vi "Write Sample Metadata.vi"(0 "File Path":path, 11 "Error In":errorcluster) -> (4 "File Path (Dup)":path, 8 "Canceled?":bool, 15 "Write Error":errorcluster)   [LabVIEW 2016]
uses:
  <vilib>/Utility/miscctls.llb/LVPointTypeDef.ctl
  Sampel Metadata Type Defs/Sample Metadata Full Data.ctl
  Sampel Metadata Type Defs/Sample Metadata Name Value Pair.ctl
  Sampel Metadata Type Defs/Sample Metadata Probe Data.ctl
  <vilib>/regexp/Match Regular Expression.xnode
  shell32.dll
panel:
  in  "Abort":bool
  in  "User Name":u16(ring) items=["Not Applicable", "-", "Add Item"]
  out "Current Path":string
  out "Last File Write Error":errorcluster
  in  "Dirty Quit":bool
  in  "Scavenger 06":u16(ring) items=["Not Applicable", "-", "Add Item"]
  in  "Scavenger 05":u16(ring) items=["Not Applicable", "-", "Add Item"]
  in  "Scavenger 04":u16(ring) items=["Not Applicable", "-", "Add Item"]
  in  "Scavenger 03":u16(ring) items=["Not Applicable", "-", "Add Item"]
  in  "Scavenger 02":u16(ring) items=["Not Applicable", "-", "Add Item"]
  in  "Scavenger 01":u16(ring) items=["Not Applicable", "-", "Add Item"]
  in  "Load Preset":bool
  in  "Sealant":u16(ring) items=["Not Applicable", "-", "Add Item"]
  in  "Sample Holder":u16(ring) items=["Not Applicable", "-", "Add Item"]
  in  "Preset Metadata":u16(ring) items=["None"]
  in  "Save New Preset":bool
  in  "Notes":string caption="Additional Notes (e.g. fixation info)"
  in  "Extra Tag 06":u16(ring) caption="Extra Tag" items=["Not Applicable", "-", "Add Item"]
  in  "Extra Tag 05":u16(ring) caption="Extra Tag" items=["Not Applicable", "-", "Add Item"]
  in  "Extra Tag 04":u16(ring) caption="Extra Tag" items=["Not Applicable", "-", "Add Item"]
  in  "Extra Tag 03":u16(ring) caption="Extra Tag" items=["Not Applicable", "-", "Add Item"]
  in  "Extra Tag 02":u16(ring) caption="Extra Tag" items=["Not Applicable", "-", "Add Item"]
  in  "Extra Tag 01":u16(ring) caption="Extra Tag" items=["Not Applicable", "-", "Add Item"]
  in  "Image Target 04":u16(ring) caption="Image Target" items=["Not Applicable", "-", "Add Item"]
  in  "Image Target 03":u16(ring) caption="Image Target" items=["Not Applicable", "-", "Add Item"]
  in  "Image Target 02":u16(ring) caption="Image Target" items=["Not Applicable", "-", "Add Item"]
  in  "Image Target 01":u16(ring) caption="Probe Target" items=["Not Applicable", "-", "Add Item"]
  in  "Buffer PH":dbl=1.0 caption="PH"
  in  "Buffer Type":u16(ring) items=["Not Applicable", "-", "Add Item"]
  in  "Probe Concentration 04":dbl=1.0 caption="Concentration"
  in  "Probe Concentration 03":dbl=1.0 caption="Concentration"
  in  "Probe Concentration 02":dbl=1.0 caption="Concentration"
  in  "Probe Concentration 01":dbl=1.0 caption="Concentration"
  in  "Probe Cat Num 04":u16(ring) caption="Probe Cat Num" items=["Not Applicable", "-", "Add Item"]
  in  "Probe Sub Type 04":u16(ring) caption="Probe Sub Type" items=["Not Applicable", "-", "Add Item"]
  in  "Probe Name 04":u16(ring) caption="Probe Name" items=["Not Applicable", "-", "Add Item"]
  in  "Probe 4":bool
  in  "Probe Cat Num 03":u16(ring) caption="Probe Cat Num" items=["Not Applicable", "-", "Add Item"]
  in  "Probe Cat Num 02":u16(ring) caption="Probe Cat Num" items=["Not Applicable", "-", "Add Item"]
  in  "Probe Cat Num 01":u16(ring) caption="Catalog Number" items=["Not Applicable", "-", "Add Item"]
  in  "Probe Sub Type 03":u16(ring) caption="Probe Sub Type" items=["Not Applicable", "-", "Add Item"]
  in  "Probe Sub Type 02":u16(ring) caption="Probe Sub Type" items=["Not Applicable", "-", "Add Item"]
  in  "Probe Sub Type 01":u16(ring) caption="Probe Sub Type" items=["Not Applicable", "-", "Add Item"]
  in  "Probe Name 03":u16(ring) caption="Probe Name" items=["Not Applicable", "-", "Add Item"]
  in  "Probe Name 02":u16(ring) caption="Probe Name" items=["Not Applicable", "-", "Add Item"]
  in  "Probe Name 01":u16(ring) caption="Probe Name" items=["Not Applicable", "-", "Add Item"]
  in  "Probe 3":bool
  in  "Probe 2":bool
  in  "Probe 1":bool
  in  "Sample Type Sub Types":u16(ring) caption="Sample Sub Type" items=["Not Applicable", "-", "Add Item"]
  in  "Sample Type":u16(ring) items=["Not Applicable", "-", "Add Item"]
  in  "Cancel":bool
  in  "Save":bool
  # "Sample Type"
  # "Sample Mounting"
  # "Buffer Information"
  # "Oxygen Scavenger Components"
  # "Probe Information"
  # "Probe Active"
  # "Additional Tags"
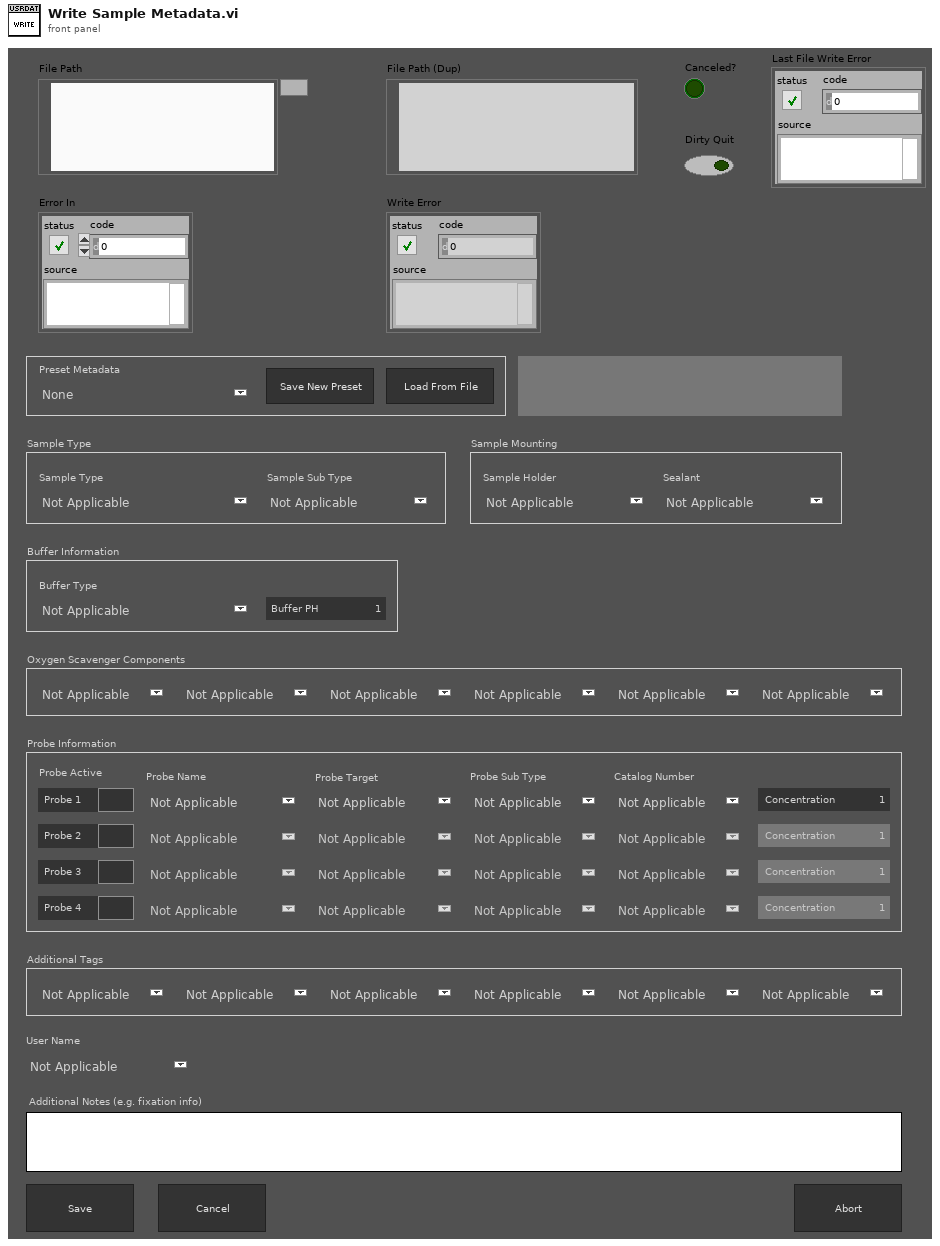
[diagram p1: front panel]
types:
  T1 = typedef "Sample Metadata Full Data.ctl" = cluster{"Sample Type":T2, "Sample Sub Type":T2, "Proble Data":T3[], "Buffer Type":T2, "Buffer PH":dbl, "Extra Tags":T2[], "Sample Holder":T2, "Sealant":T2, "Notes":string, "Preset Name":string, "Scavenger Tags":T2[], "User Name":T2}
  T2 = typedef "Sample Metadata Name Value Pair.ctl" = cluster{"String":string, "Value":u16}
  T3 = typedef "Sample Metadata Probe Data.ctl" = cluster{"Active?":bool, "Name":T2, "Target":T2, "Sub Type":T2, "Cat Number":T2, "Concentration":dbl}
  T4 = enum16{"Always On", "Always Off", "Off While Running"}
  T5 = typedef "LVPointTypeDef.ctl" = cluster{"Horizontal":i16, "Vertical":i16}
  T6 = enum8{"Enabled", "Disabled", "Disabled and Grayed Out"}
  T7 = typedef "LVRectTypeDef.ctl" = cluster{"Left":i16, "Top":i16, "Right":i16, "Bottom":i16}
  T8 = typedef "LVBoundsTypeDef.ctl" = cluster{"Width":u32, "Height":u32}
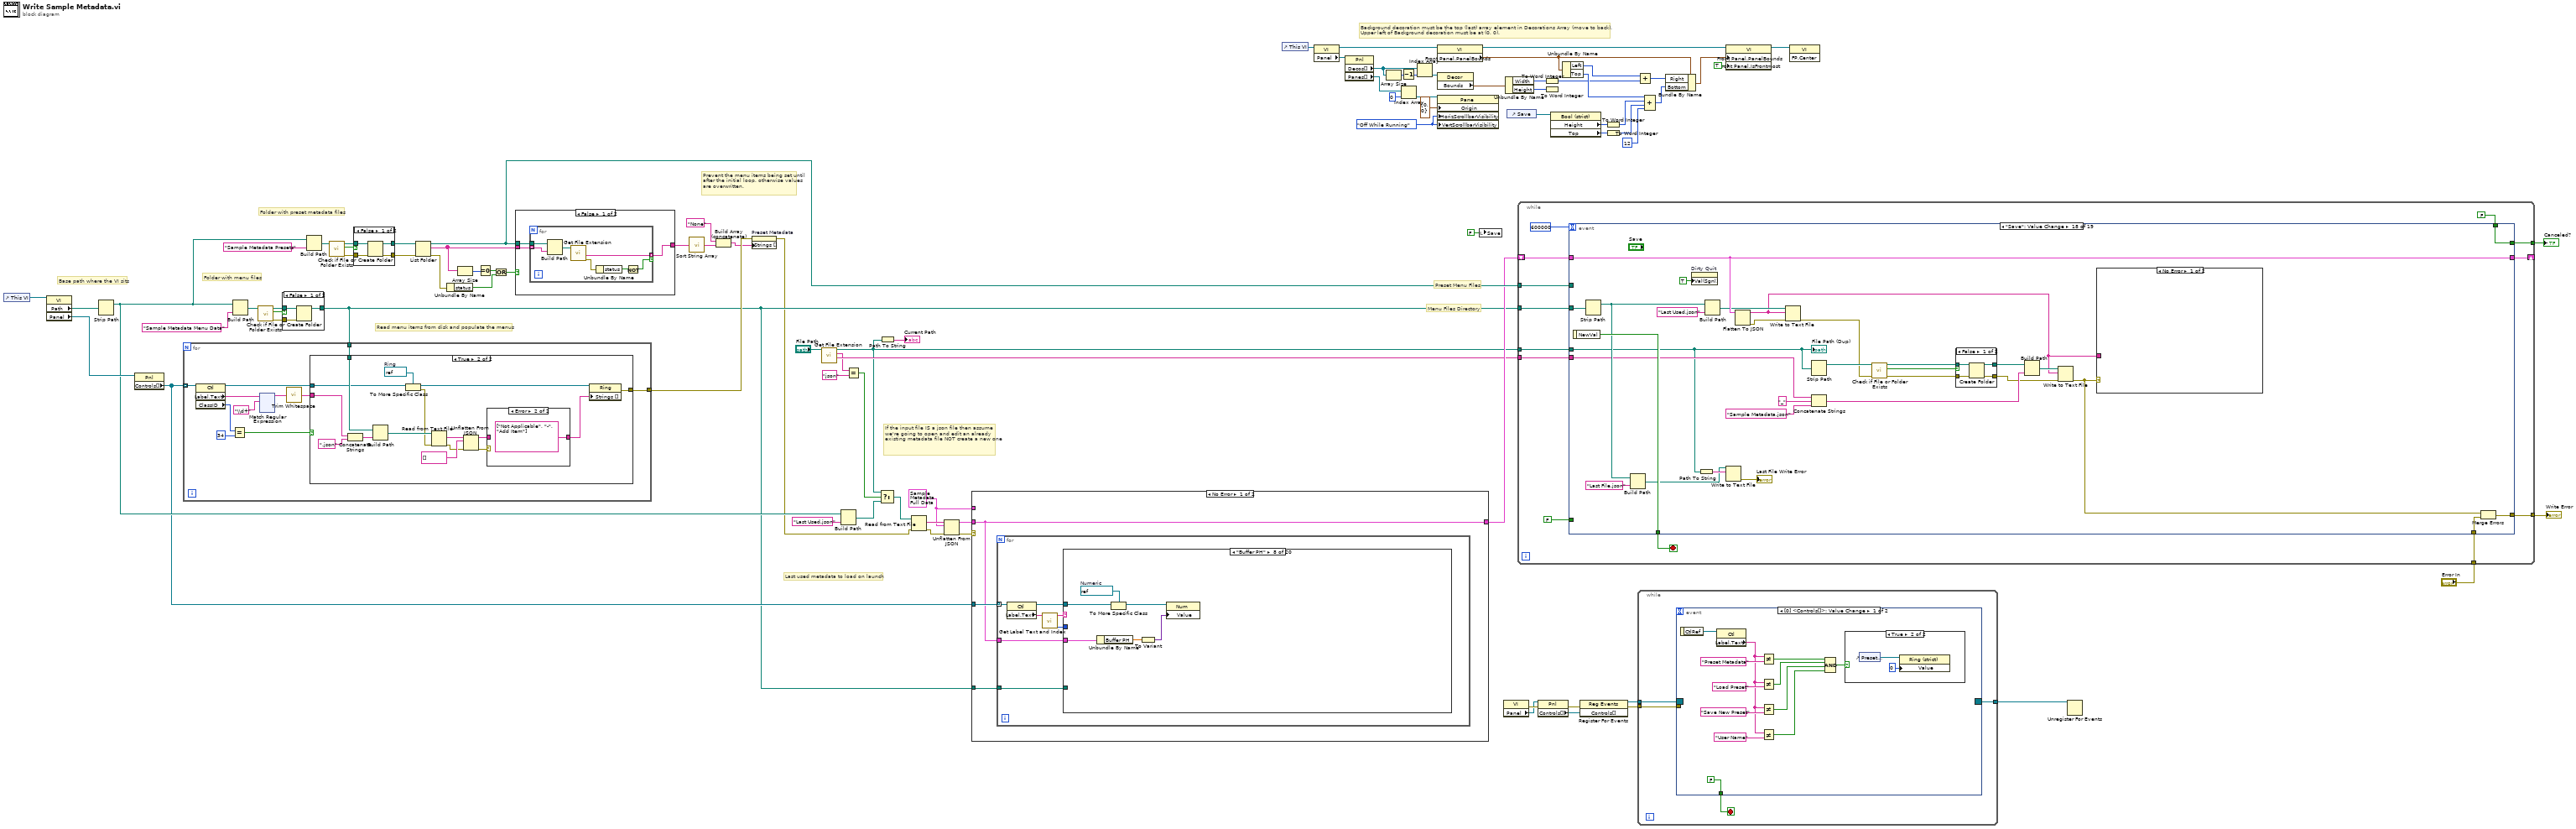
[diagram p0: block diagram]
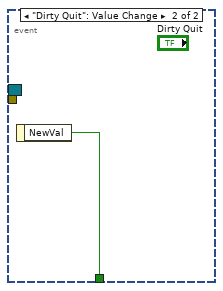
[diagram p3: hidden frame]
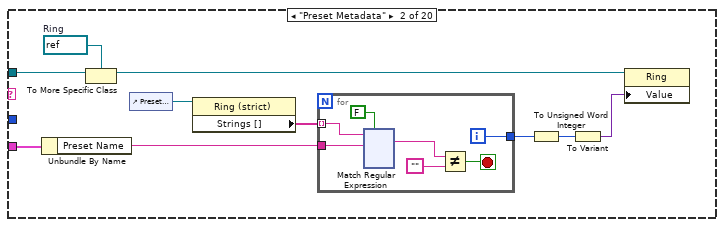
[diagram p5: hidden frame]
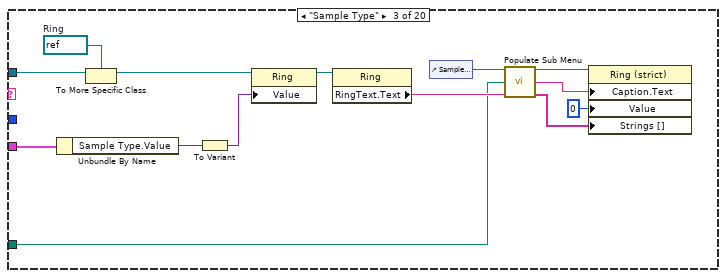
[diagram p6: hidden frame]
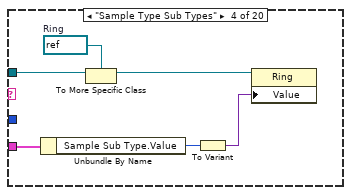
[diagram p7: hidden frame]
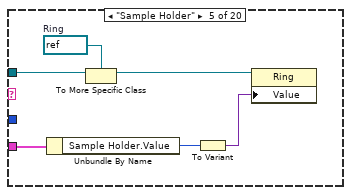
[diagram p8: hidden frame]
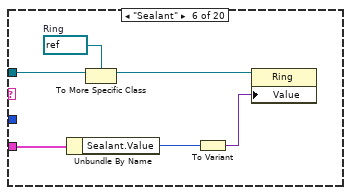
[diagram p9: hidden frame]
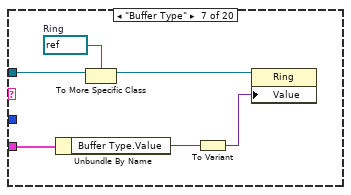
[diagram p10: hidden frame]
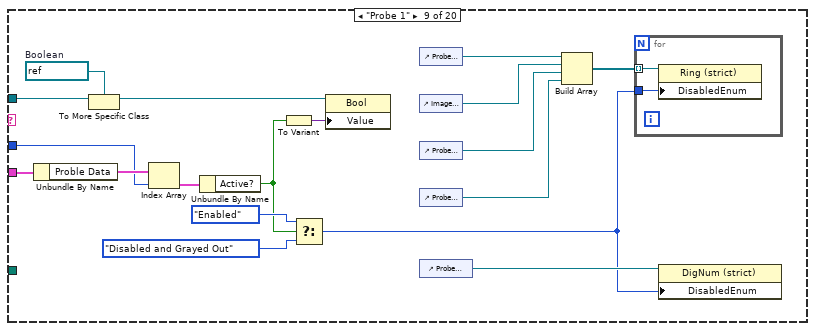
[diagram p11: hidden frame]
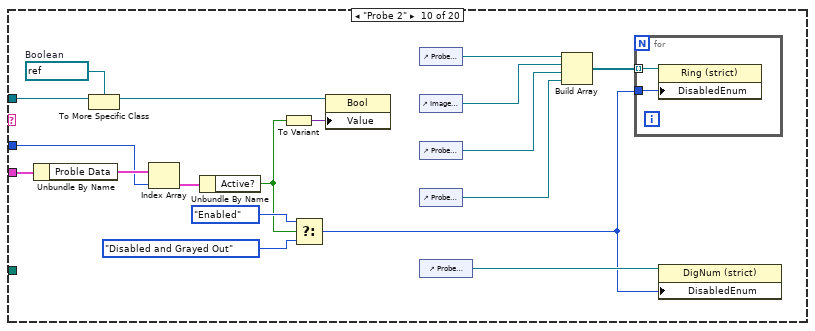
[diagram p12: hidden frame]
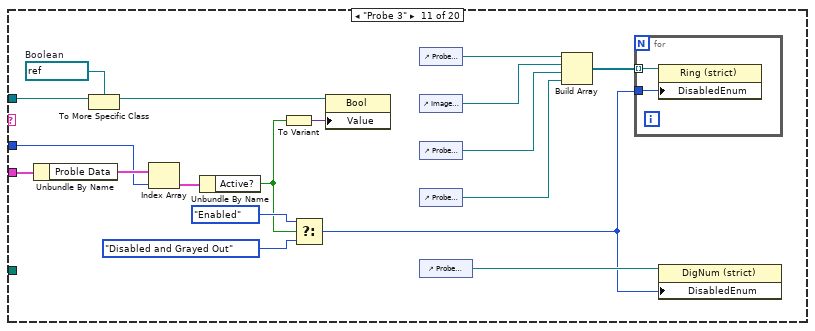
[diagram p13: hidden frame]
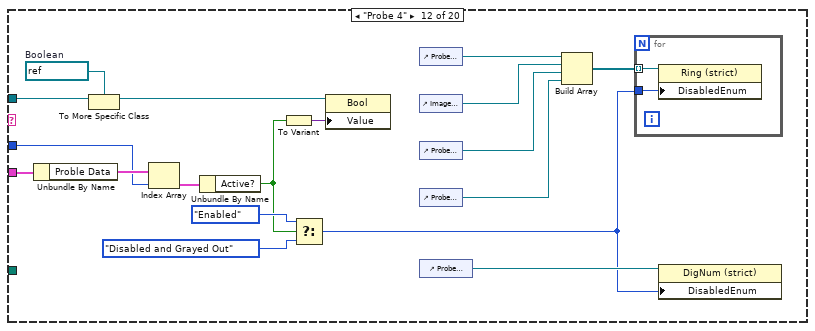
[diagram p14: hidden frame]
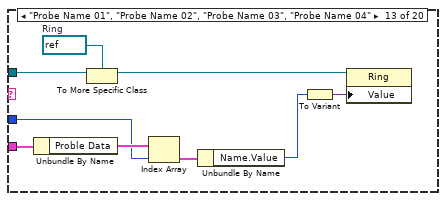
[diagram p15: hidden frame]
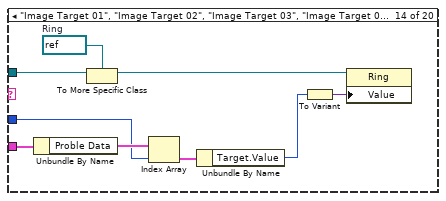
[diagram p16: hidden frame]
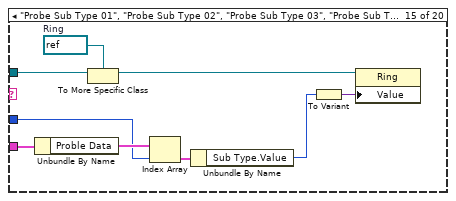
[diagram p17: hidden frame]
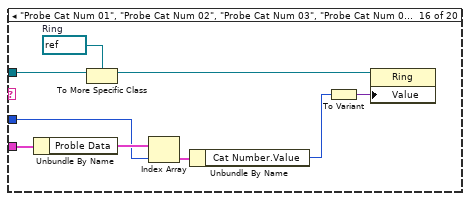
[diagram p18: hidden frame]
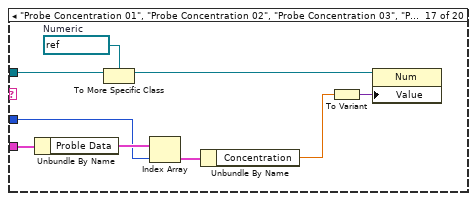
[diagram p19: hidden frame]
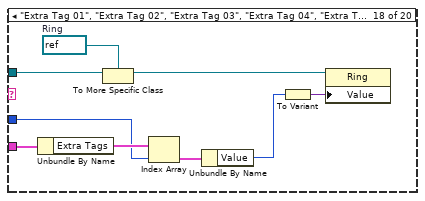
[diagram p20: hidden frame]
diagram:
  w30 = T1 {"Sample Type"={"String"="", "Value"=0}, "Sample Sub Type"={"String"="", "Value"=0}, "Proble Data"=[{"Active?"=FALSE, "Name"={"String"="", "Value"=0}, "Target"={"String"="", "Value"=0}, "Sub Type"={"String"="", "Value"=0}, "Cat Number"={"String"="", "Value"=0}, "Concentration"=0.0}, {"Active?"=FALSE, "Name"={"String"="", "Value"=0}, "Target"={"String"="", "Value"=0}, "Sub Type"={"String"="", "Value"=0}, "Cat Number"={"String"="", "Value"=0}, "Concentration"=0.0}, {"Active?"=FALSE, "Name"={"String"="", "Value"=0}, "Target"={"String"="", "Value"=0}, "Sub Type"={"String"="", "Value"=0}, "Cat Number"={"String"="", "Value"=0}, "Concentration"=0.0}, {"Active?"=FALSE, "Name"={"String"="", "Value"=0}, "Target"={"String"="", "Value"=0}, "Sub Type"={"String"="", "Value"=0}, "Cat Number"={"String"="", "Value"=0}, "Concentration"=0.0}], "Buffer Type"={"String"="", "Value"=0}, "Buffer PH"=0.0, "Extra Tags"=[{"String"="", "Value"=0}, {"String"="", "Value"=0}, {"String"="", "Value"=0}, {"String"="", "Value"=0}, {"String"="", "Value"=0}, {"String"="", "Value"=0}], "Sample Holder"={"String"="", "Value"=0}, "Sealant"={"String"="", "Value"=0}, "Notes"="", "Preset Name"="", "Scavenger Tags"=[{"String"="", "Value"=0}, {"String"="", "Value"=0}, {"String"="", "Value"=0}, {"String"="", "Value"=0}, {"String"="", "Value"=0}, {"String"="", "Value"=0}], "User Name"={"String"="", "Value"=0}} ("Sample Metadata")
  w72 = T4."Off While Running" ("Vertical Scrollbar Visibility")
  # "If the input file IS a json file then assume we're going to open and edit an already existing metadata file NOT create a new one"
  # "Last used metadata to load on launch"
  # "Preset Menu Files"
  # "Menu Files Directory"
  # "Prevent the menu items being set until after the initial loop, otherwise values are overwritten."
  # "Folder with preset metadata files"
  # "Folder with menu files"
  # "Read menu items from disk and populate the menus"
  # "Base path where the VI sits"
  # "Background decoration must be the top (last) array element in Decorations Array (move to back).\nUpper left of Background decoration must be at (0, 0)."
  n1 = control-ref of="This VI"() -> (w58:refnum<vi>)
  n2 = property class="VI"(reference=w58) -> ("Path"=w35:path, "Panel"=w56:refnum<vi>)  [unwired: 1 in, 2 out]
  n3 = Strip Path(path=w35) -> (stripped path=w34:path)  [unwired: 1 out]
  n4 = property class="Pnl"(reference=w56) -> ("Controls[]"=w29:refnum<vi>[])  [unwired: 1 in, 2 out]
  n5 = Build Path(base path=w34, name or relative path="Sample Metadata Menu Data") -> (appended path=w54:path)
  n6 = call <vilib>:"Check if File or Folder Exists.vi"("path"=w54) -> ("error out"=w39:errorcluster, "file or folder exists?"=w52:bool, "dup path"=w53:path)  [unwired: 8 in]
  n7 = case shown="False" w52 {
    tunnel: w53 -> [w92 w93]
    tunnel: [w91 w93] -> w27
    tunnel: w39 -> [w90 _]
    frame False {
      n8 = Create Folder(path (use dialog)=w92, error in=w90) -> (created path=w91:path)  [unwired: 1 in, 2 out]
    }
    frame True {
    }
  }
  n9 = for {
    tunnel: w29 -> [w104] mode=indexing
    tunnel: w27 -> [w100]
    tunnel: [w94] -> w38
    n10 = property class="Ctl"(reference=w104) -> (reference out=w102:refnum<vi>, "Label.Text"=w97:string, "ClassID"=w101:u32)  [unwired: 1 in, 1 out]
    n11 = Equal?(x=w101, y=u32 34) -> (x = y?=w103:bool)
    n12 = xnode "Match Regular Expression"("input string"=w97, "regular expression"="\\d+") -> ("before match"=w99:string)  [unwired: 4 in, 4 out]
    n13 = call <vilib>:"Trim Whitespace.vi"("string"=w99) -> ("trimmed string"=w96:string)  [unwired: 1 in]
    n14 = case shown="True" w103 {
      tunnel: w102 -> [_ w225]
      tunnel: w96 -> [_ w233]
      tunnel: w100 -> [_ w232]
      tunnel: [errorcluster {"status"=FALSE, "code"=0, "source"=""} ("error out") w220] -> w94
      frame False {
      }
      frame True {
        w224 = refnum<vi> refnum  # Ring
        n15 = Concatenate Strings(w233, ".json") -> (w234:string)
        n16 = Build Path(base path=w232, name or relative path=w234) -> (appended path=w231:path)
        n17 = To More Specific Class(target class=w224, reference=w225) -> (specific class reference=w223:refnum<vi>, error out=w221:errorcluster)  [unwired: 1 in]
        n18 = Read from Text File(file (use dialog)=w231, error in=w221) -> (text=w230:string, error out=w228:errorcluster)  [unwired: 2 in, 2 out]
        n19 = Unflatten From JSON(JSON string=w230, type and defaults=string[] [], error in (no error)=w228) -> (value=w226:string[], error out=w227:errorcluster)  [unwired: 4 in]
        n20 = case shown="Error" w227 {
          tunnel: w226 -> [w236 _]
          tunnel: [w236 string[] ["Not Applicable", "-", "Add Item"]] -> w222
          frame No Error {
          }
          frame Error {
          }
        }
        n21 = property class="Ring"(reference=w223, "Strings []"=w222) -> (error out=w220:errorcluster)  [unwired: 1 in, 1 out]
      }
    }
  }
  n22 = Build Path(base path=w34, name or relative path="Sample Metadata Presets") -> (appended path=w49:path)
  n23 = call <vilib>:"Check if File or Folder Exists.vi"("path"=w49) -> ("error out"=w41:errorcluster, "file or folder exists?"=w51:bool, "dup path"=w50:path)  [unwired: 8 in]
  n24 = case shown="False" w51 {
    tunnel: w50 -> [w241 w243]
    tunnel: [w240 w243] -> w48
    tunnel: w41 -> [w239 w242]
    tunnel: [w238 w242] -> w40
    frame False {
      n25 = Create Folder(path (use dialog)=w241, error in=w239) -> (created path=w240:path, error out=w238:errorcluster)  [unwired: 1 in, 1 out]
    }
    frame True {
    }
  }
  n26 = List Folder(path=w48, error in=w40) -> (path out=w37:path, filenames=w46:string[], error out=w47:errorcluster)  [unwired: 2 in, 1 out]
  n27 = Unbundle By Name(w47) -> ("status"=w43:bool)
  n28 = Array Size(array=w46) -> (size(s)=w45:i32)
  n29 = Equal To 0?(x=w45) -> (x = 0?=w44:bool)
  n30 = Or(x=w44, y=w43) -> (x .or. y?=w42:bool)
  n31 = case shown="False" w42 {
    tunnel: w46 -> [w246 _]
    tunnel: [w244 string[] []] -> w23
    tunnel: w37 -> [w245 _]
    frame False {
      n32 = for {
        tunnel: w246 -> [w252] mode=indexing
        tunnel: w245 -> [w253]
        tunnel: [w250] -> w244 mode=indexing if=w247
        n33 = Build Path(base path=w253, name or relative path=w252) -> (appended path=w251:path)
        n34 = call <vilib>:"Get File Extension.vi"("file"=w251) -> ("error out"=w249:errorcluster, "filename without extension"=w250:string)  [unwired: 6 in, 3 out]
        n35 = Unbundle By Name(w249) -> ("status"=w248:bool)
        n36 = Not(x=w248) -> (.not. x?=w247:bool)
      }
    }
    frame True {
    }
  }
  n37 = call "Sort String Array.vi"("Array of String"=w23) -> ("Sorted Array"=w22:string[])  [unwired: 14 in]
  n38 = Build Array (concatenate)("None", w22) -> (w20:string[])
  n39 = property on="Preset Metadata" class="Ring (strict)"(error in=w38, "Strings []"=w20) -> (error out=w19:errorcluster)  [unwired: 1 in, 1 out]
  n40 = call <vilib>:"Get File Extension.vi"("file"="File Path") -> ("filename without extension"=w9:string, "lowercase file extension"=w8:string, "dup file"=w3:path)  [unwired: 6 in, 2 out]
  n41 = Build Path(base path=w34, name or relative path="Last Used.json") -> (appended path=w5:path)
  n42 = Equal?(x=w8, y="json") -> (x = y?=w6:bool)
  n43 = Select(t=w3, s=w6, f=w5) -> (s? t:f=w4:path)
  n44 = Path To String(path=w3) -> (string=→"Current Path":string)
  n45 = Read from Text File(file (use dialog)=w4, error in=w19) -> (text=w33:string, error out=w18:errorcluster)  [unwired: 2 in, 2 out]
  n46 = Unflatten From JSON(JSON string=w33, type and defaults=w30, error in (no error)=w18) -> (value=w31:T1, error out=w32:errorcluster)  [unwired: 4 in]
  n47 = case shown="No Error" w32 {
    tunnel: [w255 w597] -> w28
    tunnel: w29 -> [w257 _]
    tunnel: w27 -> [w256 w589]
    tunnel: w31 -> [w255 _]
    tunnel: w30 -> [_ w597]
    frame No Error {
      n48 = for {
        tunnel: w257 -> [w264] mode=indexing
        tunnel: w255 -> [w262]
        tunnel: w256 -> [w261]
        n49 = property class="Ctl"(reference=w264) -> (reference out=w263:refnum<vi>, "Label.Text"=w260:string)  [unwired: 1 in, 1 out]
        n50 = call "Get Label Text and Index.vi"("Label Text and Index"=w260) -> ("Label Text and Index (Dup)"=w259:string, "Index"=w258:i32)  [unwired: 12 in, 1 out]
        n51 = case shown="\"Buffer PH\"" w259 {
          tunnel: w263 -> [_ w273 w408 w414 w420 w426 w432 w438 w453 w473 w493 w513 w525 w534 w543 w552 w561 w570 w579 w585]
          tunnel: w262 -> [_ w271 w406 w412 w418 w424 w430 w436 w457 w477 w497 w517 w528 w537 w546 w555 w564 w573 w582 w584]
          tunnel: w261 -> [_ _ w396 _ _ _ _ _ _ _ _ _ _ _ _ _ _ _ _ _]
          tunnel: w258 -> [_ _ _ _ _ _ _ _ w440 w460 w480 w500 w520 w529 w538 w547 w556 w565 w574 _]
          frame Default {
          }
          frame "Preset Metadata" {
            w274 = refnum<vi> refnum  # Ring
            n52 = Unbundle By Name(w271) -> ("Preset Name"=w266:string)
            n53 = To More Specific Class(target class=w274, reference=w273) -> (specific class reference=w272:refnum<vi>)  [unwired: 1 in, 1 out]
            n54 = control-ref of="Preset Metadata"() -> (w268:refnum<vi>)
            n55 = property class="Ring (strict)"(reference=w268) -> ("Strings []"=w269:string[])  [unwired: 1 in, 2 out]
            n56 = for {
              tunnel: w266 -> [w281]
              tunnel: w269 -> [w279] mode=indexing
              tunnel: [w275] -> w267
              i -> [w275]
              stop <- w278 stop-if-true
              n57 = xnode "Match Regular Expression"("input string"=w279, "regular expression"=w281, "ignore case? (F)"=FALSE) -> ("whole match"=w277:string)  [unwired: 3 in, 4 out]
              n58 = Not Equal?(x=w277, y="") -> (x != y?=w278:bool)
            }
            n59 = To Unsigned Word Integer(number=w267) -> (unsigned 16bit integer=w265:u16)
            n60 = To Variant(anything=w265) -> (Variant=w270:variant)
            n61 = property class="Ring"(reference=w272, "Value"=w270) -> ()  [unwired: 1 in, 2 out]
          }
          frame "Sample Type" {
            w409 = refnum<vi> refnum  # Ring
            n62 = Unbundle By Name(w406) -> ("Sample Type.Value"=w405:u16)
            n63 = To More Specific Class(target class=w409, reference=w408) -> (specific class reference=w407:refnum<vi>)  [unwired: 1 in, 1 out]
            n64 = To Variant(anything=w405) -> (Variant=w404:variant)
            n65 = property class="Ring"(reference=w407, "Value"=w404) -> (reference out=w403:refnum<vi>)  [unwired: 1 in, 1 out]
            n66 = property class="Ring"(reference=w403) -> ("RingText.Text"=w397:string)  [unwired: 1 in, 2 out]
            n67 = control-ref of="Sample Type Sub Types"() -> (w401:refnum<vi>)
            n68 = call "Populate Sub Menu.vi"("Sample Type Sub Types"=w401, "Base Path"=w396, "Ring Text"=w397) -> ("Sample Type Sub Types (Dup)"=w400:refnum<vi>, "Caption Text"=w399:string, "Menu Items"=w398:string[])  [unwired: 10 in]
            n69 = property class="Ring (strict)"(reference=w400, "Caption.Text"=w399, "Value"=u16 0, "Strings []"=w398) -> ()  [unwired: 1 in, 2 out]
          }
          frame "Sample Type Sub Types" {
            w415 = refnum<vi> refnum  # Ring
            n70 = Unbundle By Name(w412) -> ("Sample Sub Type.Value"=w411:u16)
            n71 = To More Specific Class(target class=w415, reference=w414) -> (specific class reference=w413:refnum<vi>)  [unwired: 1 in, 1 out]
            n72 = To Variant(anything=w411) -> (Variant=w410:variant)
            n73 = property class="Ring"(reference=w413, "Value"=w410) -> ()  [unwired: 1 in, 2 out]
          }
          frame "Sample Holder" {
            w421 = refnum<vi> refnum  # Ring
            n74 = Unbundle By Name(w418) -> ("Sample Holder.Value"=w417:u16)
            n75 = To More Specific Class(target class=w421, reference=w420) -> (specific class reference=w419:refnum<vi>)  [unwired: 1 in, 1 out]
            n76 = To Variant(anything=w417) -> (Variant=w416:variant)
            n77 = property class="Ring"(reference=w419, "Value"=w416) -> ()  [unwired: 1 in, 2 out]
          }
          frame "Sealant" {
            w427 = refnum<vi> refnum  # Ring
            n78 = Unbundle By Name(w424) -> ("Sealant.Value"=w423:u16)
            n79 = To More Specific Class(target class=w427, reference=w426) -> (specific class reference=w425:refnum<vi>)  [unwired: 1 in, 1 out]
            n80 = To Variant(anything=w423) -> (Variant=w422:variant)
            n81 = property class="Ring"(reference=w425, "Value"=w422) -> ()  [unwired: 1 in, 2 out]
          }
          frame "Buffer Type" {
            w433 = refnum<vi> refnum  # Ring
            n82 = Unbundle By Name(w430) -> ("Buffer Type.Value"=w429:u16)
            n83 = To More Specific Class(target class=w433, reference=w432) -> (specific class reference=w431:refnum<vi>)  [unwired: 1 in, 1 out]
            n84 = To Variant(anything=w429) -> (Variant=w428:variant)
            n85 = property class="Ring"(reference=w431, "Value"=w428) -> ()  [unwired: 1 in, 2 out]
          }
          frame "Buffer PH" {
            w439 = refnum<vi> refnum  # Numeric
            n86 = Unbundle By Name(w436) -> ("Buffer PH"=w435:dbl)
            n87 = To More Specific Class(target class=w439, reference=w438) -> (specific class reference=w437:refnum<vi>)  [unwired: 1 in, 1 out]
            n88 = To Variant(anything=w435) -> (Variant=w434:variant)
            n89 = property class="Num"(reference=w437, "Value"=w434) -> ()  [unwired: 1 in, 2 out]
          }
          frame "Probe 1" {
            w454 = refnum<vi> refnum  # Boolean
            n90 = Unbundle By Name(w457) -> ("Proble Data"=w456:T3[])
            n91 = To More Specific Class(target class=w454, reference=w453) -> (specific class reference=w452:refnum<vi>)  [unwired: 1 in, 1 out]
            n92 = Index Array(array=w456, index=w440) -> (element=w455:T3)
            n93 = Unbundle By Name(w455) -> ("Active?"=w442:bool)
            n94 = To Variant(anything=w442) -> (Variant=w451:variant)
            n95 = Select(t=T6."Enabled" ("Disabled"), s=w442, f=T6."Disabled and Grayed Out" ("Disabled")) -> (s? t:f=w441:T6)
            n96 = property class="Bool"(reference=w452, "Value"=w451) -> ()  [unwired: 1 in, 2 out]
            n97 = control-ref of="Probe Name 01"() -> (w447:refnum<vi>)
            n98 = control-ref of="Image Target 01"() -> (w448:refnum<vi>)
            n99 = control-ref of="Probe Sub Type 01"() -> (w449:refnum<vi>)
            n100 = control-ref of="Probe Cat Num 01"() -> (w450:refnum<vi>)
            n101 = control-ref of="Probe Concentration 01"() -> (w445:refnum<vi>)
            n102 = Build Array(w447, w448, w449, w450) -> (w446:refnum<vi>[])
            n103 = for {
              tunnel: w446 -> [w459] mode=indexing
              tunnel: w441 -> [w458]
              n104 = property class="Ring (strict)"(reference=w459, "DisabledEnum"=w458) -> ()  [unwired: 1 in, 2 out]
            }
            n105 = property class="DigNum (strict)"(reference=w445, "DisabledEnum"=w441) -> ()  [unwired: 1 in, 2 out]
          }
          frame "Probe 2" {
            w474 = refnum<vi> refnum  # Boolean
            n106 = Unbundle By Name(w477) -> ("Proble Data"=w476:T3[])
            n107 = To More Specific Class(target class=w474, reference=w473) -> (specific class reference=w472:refnum<vi>)  [unwired: 1 in, 1 out]
            n108 = Index Array(array=w476, index=w460) -> (element=w475:T3)
            n109 = Unbundle By Name(w475) -> ("Active?"=w462:bool)
            n110 = To Variant(anything=w462) -> (Variant=w471:variant)
            n111 = Select(t=T6."Enabled" ("Disabled"), s=w462, f=T6."Disabled and Grayed Out" ("Disabled")) -> (s? t:f=w461:T6)
            n112 = property class="Bool"(reference=w472, "Value"=w471) -> ()  [unwired: 1 in, 2 out]
            n113 = control-ref of="Probe Name 02"() -> (w467:refnum<vi>)
            n114 = control-ref of="Image Target 02"() -> (w468:refnum<vi>)
            n115 = control-ref of="Probe Sub Type 02"() -> (w469:refnum<vi>)
            n116 = control-ref of="Probe Cat Num 02"() -> (w470:refnum<vi>)
            n117 = control-ref of="Probe Concentration 02"() -> (w465:refnum<vi>)
            n118 = Build Array(w467, w468, w469, w470) -> (w466:refnum<vi>[])
            n119 = for {
              tunnel: w466 -> [w479] mode=indexing
              tunnel: w461 -> [w478]
              n120 = property class="Ring (strict)"(reference=w479, "DisabledEnum"=w478) -> ()  [unwired: 1 in, 2 out]
            }
            n121 = property class="DigNum (strict)"(reference=w465, "DisabledEnum"=w461) -> ()  [unwired: 1 in, 2 out]
          }
          frame "Probe 3" {
            w494 = refnum<vi> refnum  # Boolean
            n122 = Unbundle By Name(w497) -> ("Proble Data"=w496:T3[])
            n123 = To More Specific Class(target class=w494, reference=w493) -> (specific class reference=w492:refnum<vi>)  [unwired: 1 in, 1 out]
            n124 = Index Array(array=w496, index=w480) -> (element=w495:T3)
            n125 = Unbundle By Name(w495) -> ("Active?"=w482:bool)
            n126 = To Variant(anything=w482) -> (Variant=w491:variant)
            n127 = Select(t=T6."Enabled" ("Disabled"), s=w482, f=T6."Disabled and Grayed Out" ("Disabled")) -> (s? t:f=w481:T6)
            n128 = property class="Bool"(reference=w492, "Value"=w491) -> ()  [unwired: 1 in, 2 out]
            n129 = control-ref of="Probe Name 03"() -> (w487:refnum<vi>)
            n130 = control-ref of="Image Target 03"() -> (w488:refnum<vi>)
            n131 = control-ref of="Probe Sub Type 03"() -> (w489:refnum<vi>)
            n132 = control-ref of="Probe Cat Num 03"() -> (w490:refnum<vi>)
            n133 = control-ref of="Probe Concentration 03"() -> (w485:refnum<vi>)
            n134 = Build Array(w487, w488, w489, w490) -> (w486:refnum<vi>[])
            n135 = for {
              tunnel: w486 -> [w499] mode=indexing
              tunnel: w481 -> [w498]
              n136 = property class="Ring (strict)"(reference=w499, "DisabledEnum"=w498) -> ()  [unwired: 1 in, 2 out]
            }
            n137 = property class="DigNum (strict)"(reference=w485, "DisabledEnum"=w481) -> ()  [unwired: 1 in, 2 out]
          }
          frame "Probe 4" {
            w514 = refnum<vi> refnum  # Boolean
            n138 = Unbundle By Name(w517) -> ("Proble Data"=w516:T3[])
            n139 = To More Specific Class(target class=w514, reference=w513) -> (specific class reference=w512:refnum<vi>)  [unwired: 1 in, 1 out]
            n140 = Index Array(array=w516, index=w500) -> (element=w515:T3)
            n141 = Unbundle By Name(w515) -> ("Active?"=w502:bool)
            n142 = To Variant(anything=w502) -> (Variant=w511:variant)
            n143 = Select(t=T6."Enabled" ("Disabled"), s=w502, f=T6."Disabled and Grayed Out" ("Disabled")) -> (s? t:f=w501:T6)
            n144 = property class="Bool"(reference=w512, "Value"=w511) -> ()  [unwired: 1 in, 2 out]
            n145 = control-ref of="Probe Name 04"() -> (w507:refnum<vi>)
            n146 = control-ref of="Image Target 04"() -> (w508:refnum<vi>)
            n147 = control-ref of="Probe Sub Type 04"() -> (w509:refnum<vi>)
            n148 = control-ref of="Probe Cat Num 04"() -> (w510:refnum<vi>)
            n149 = control-ref of="Probe Concentration 04"() -> (w505:refnum<vi>)
            n150 = Build Array(w507, w508, w509, w510) -> (w506:refnum<vi>[])
            n151 = for {
              tunnel: w506 -> [w519] mode=indexing
              tunnel: w501 -> [w518]
              n152 = property class="Ring (strict)"(reference=w519, "DisabledEnum"=w518) -> ()  [unwired: 1 in, 2 out]
            }
            n153 = property class="DigNum (strict)"(reference=w505, "DisabledEnum"=w501) -> ()  [unwired: 1 in, 2 out]
          }
          frame "Probe Name 01", "Probe Name 02", "Probe Name 03", "Probe Name 04" {
            w521 = refnum<vi> refnum  # Ring
            n154 = Unbundle By Name(w528) -> ("Proble Data"=w527:T3[])
            n155 = To More Specific Class(target class=w521, reference=w525) -> (specific class reference=w524:refnum<vi>)  [unwired: 1 in, 1 out]
            n156 = Index Array(array=w527, index=w520) -> (element=w526:T3)
            n157 = Unbundle By Name(w526) -> ("Name.Value"=w522:u16)
            n158 = To Variant(anything=w522) -> (Variant=w523:variant)
            n159 = property class="Ring"(reference=w524, "Value"=w523) -> ()  [unwired: 1 in, 2 out]
          }
          frame "Image Target 01", "Image Target 02", "Image Target 03", "Image Target 04" {
            w530 = refnum<vi> refnum  # Ring
            n160 = Unbundle By Name(w537) -> ("Proble Data"=w536:T3[])
            n161 = To More Specific Class(target class=w530, reference=w534) -> (specific class reference=w533:refnum<vi>)  [unwired: 1 in, 1 out]
            n162 = Index Array(array=w536, index=w529) -> (element=w535:T3)
            n163 = Unbundle By Name(w535) -> ("Target.Value"=w531:u16)
            n164 = To Variant(anything=w531) -> (Variant=w532:variant)
            n165 = property class="Ring"(reference=w533, "Value"=w532) -> ()  [unwired: 1 in, 2 out]
          }
          frame "Probe Sub Type 01", "Probe Sub Type 02", "Probe Sub Type 03", "Probe Sub Type 04" {
            w539 = refnum<vi> refnum  # Ring
            n166 = Unbundle By Name(w546) -> ("Proble Data"=w545:T3[])
            n167 = To More Specific Class(target class=w539, reference=w543) -> (specific class reference=w542:refnum<vi>)  [unwired: 1 in, 1 out]
            n168 = Index Array(array=w545, index=w538) -> (element=w544:T3)
            n169 = Unbundle By Name(w544) -> ("Sub Type.Value"=w540:u16)
            n170 = To Variant(anything=w540) -> (Variant=w541:variant)
            n171 = property class="Ring"(reference=w542, "Value"=w541) -> ()  [unwired: 1 in, 2 out]
          }
          frame "Probe Cat Num 01", "Probe Cat Num 02", "Probe Cat Num 03", "Probe Cat Num 04" {
            w548 = refnum<vi> refnum  # Ring
            n172 = Unbundle By Name(w555) -> ("Proble Data"=w554:T3[])
            n173 = To More Specific Class(target class=w548, reference=w552) -> (specific class reference=w551:refnum<vi>)  [unwired: 1 in, 1 out]
            n174 = Index Array(array=w554, index=w547) -> (element=w553:T3)
            n175 = Unbundle By Name(w553) -> ("Cat Number.Value"=w549:u16)
            n176 = To Variant(anything=w549) -> (Variant=w550:variant)
            n177 = property class="Ring"(reference=w551, "Value"=w550) -> ()  [unwired: 1 in, 2 out]
          }
          frame "Probe Concentration 01", "Probe Concentration 02", "Probe Concentration 03", "Probe Concentration 04" {
            w557 = refnum<vi> refnum  # Numeric
            n178 = Unbundle By Name(w564) -> ("Proble Data"=w563:T3[])
            n179 = To More Specific Class(target class=w557, reference=w561) -> (specific class reference=w560:refnum<vi>)  [unwired: 1 in, 1 out]
            n180 = Index Array(array=w563, index=w556) -> (element=w562:T3)
            n181 = Unbundle By Name(w562) -> ("Concentration"=w558:dbl)
            n182 = To Variant(anything=w558) -> (Variant=w559:variant)
            n183 = property class="Num"(reference=w560, "Value"=w559) -> ()  [unwired: 1 in, 2 out]
          }
          frame "Extra Tag 01", "Extra Tag 02", "Extra Tag 03", "Extra Tag 04", "Extra Tag 05", "Extra Tag 06" {
            w566 = refnum<vi> refnum  # Ring
            n184 = Unbundle By Name(w573) -> ("Extra Tags"=w572:T2[])
            n185 = To More Specific Class(target class=w566, reference=w570) -> (specific class reference=w569:refnum<vi>)  [unwired: 1 in, 1 out]
            n186 = Index Array(array=w572, index=w565) -> (element=w571:T2)
            n187 = Unbundle By Name(w571) -> ("Value"=w567:u16)
            n188 = To Variant(anything=w567) -> (Variant=w568:variant)
            n189 = property class="Ring"(reference=w569, "Value"=w568) -> ()  [unwired: 1 in, 2 out]
          }
          frame "Scavenger 01", "Scavenger 02", "Scavenger 03", "Scavenger 04", "Scavenger 05", "Scavenger 06" {
            w575 = refnum<vi> refnum  # Ring
            n190 = Unbundle By Name(w582) -> ("Scavenger Tags"=w581:T2[])
            n191 = To More Specific Class(target class=w575, reference=w579) -> (specific class reference=w578:refnum<vi>)  [unwired: 1 in, 1 out]
            n192 = Index Array(array=w581, index=w574) -> (element=w580:T2)
            n193 = Unbundle By Name(w580) -> ("Value"=w576:u16)
            n194 = To Variant(anything=w576) -> (Variant=w577:variant)
            n195 = property class="Ring"(reference=w578, "Value"=w577) -> ()  [unwired: 1 in, 2 out]
          }
          frame "Notes" {
            w586 = refnum<vi> refnum  # String
            n196 = Unbundle By Name(w584) -> ("Notes"=w583:string)
            n197 = To More Specific Class(target class=w586, reference=w585) -> (specific class reference=w587:refnum<vi>)  [unwired: 1 in, 1 out]
            n198 = property class="Str"(reference=w587, "Value"=w583) -> ()  [unwired: 1 in, 2 out]
          }
        }
      }
    }
    frame Error {
      # "In the unlikely event that there is no \"Last Used.json\" file but there are sample sub type files we still want to load the sub type menu items"
      n199 = control-ref of="Sample Type"() -> (w590:refnum<vi>)
      n200 = property class="Ring (strict)"(reference=w590) -> (error out=w588:errorcluster, "RingText.Text"=w591:string)  [unwired: 1 in, 1 out]
      n201 = control-ref of="Sample Type Sub Types"() -> (w595:refnum<vi>)
      n202 = call "Populate Sub Menu.vi"("Sample Type Sub Types"=w595, "Base Path"=w589, "Ring Text"=w591) -> ("Sample Type Sub Types (Dup)"=w594:refnum<vi>, "Caption Text"=w593:string, "Menu Items"=w592:string[])  [unwired: 10 in]
      n203 = property class="Ring (strict)"(reference=w594, error in=w588, "Caption.Text"=w593, "Value"=u16 0, "Strings []"=w592) -> ()  [unwired: 2 out]
    }
  }
  n204 = control-ref of="This VI"() -> (w64:refnum<vi>)
  n205 = property class="VI"(reference=w64) -> (reference out=w73:refnum<vi>, "Panel"=w65:refnum<vi>)  [unwired: 1 in, 1 out]
  n206 = property class="Pnl"(reference=w65) -> ("Decos[]"=w63:refnum<vi>[], "Panes[]"=w69:refnum<vi>[])  [unwired: 1 in, 2 out]
  n207 = Array Size(array=w63) -> (size(s)=w61:i32)
  n208 = Decrement(x=w61) -> (x-1=w62:i32)
  n209 = Index Array(array=w69, index=0) -> (element=w68:refnum<vi>)
  n210 = Index Array(array=w63, index=w62) -> (element=w71:refnum<vi>)
  n211 = property class="VI"(reference=w73) -> (reference out=w75:refnum<vi>, "Front Panel.PanelBounds"=w76:T7)  [unwired: 1 in, 1 out]
  n212 = property class="Decor"(reference=w71) -> ("Bounds"=w74:T8)  [unwired: 1 in, 2 out]
  n213 = property class="Pane"(reference=w68, "Origin"=T5 {"Horizontal"=0, "Vertical"=0}, "HorizScrollbarVisibility"=w72, "VertScrollbarVisibility"=w72) -> ()  [unwired: 1 in, 2 out]
  n214 = local write "Save"(FALSE ("Save")) -> ()
  n215 = property class="VI"() -> (error out=w17:errorcluster, "Panel"=w16:refnum<vi>)  [unwired: 2 in, 1 out]
  n216 = Unbundle By Name(w74) -> ("Width"=w79:u32, "Height"=w82:u32)
  n217 = control-ref of="Save"() -> (w66:refnum<vi>)
  n218 = while {
    tunnel: w27 -> [w609]
    shift-right: [w606] -> _
    shift-left: w28 -> [w607]
    tunnel: w37 -> [w605]
    tunnel: "Error In" -> [w603]
    tunnel: [w604] -> w25
    tunnel: [w600] -> w24
    tunnel: w3 -> [w599]
    tunnel: w9 -> [w598]
    stop <- w602 stop-if-true
    n219 = event shown="[17] \"Save\": Value Change" {
      selector: _ -> [_ _ _ _ _ _ _ _ _ _ _ _ _ _ _ _ _ _ _]
      dyn-events: _ -> [_ _ _ _ _ _ _ _ _ _ _ _ _ _ _ _ _ _ _]
      timeout: 600000 -> [_ _ _ _ _ _ _ _ _ _ _ _ _ _ _ _ _ _ _]
      tunnel: [w611 w630 w713 w749 w802 w849 w896 w943 w988 w1035 w1080 w1096 w1127 w1133 w1159 w1518 w1663 w1695 TRUE ("NewVal")] -> w602
      tunnel: w609 -> [_ w625 w708 _ w798 w845 w892 w939 w984 w1031 _ w1089 _ _ w1149 _ _ w1678 _]
      tunnel: FALSE -> [w611 w630 w713 w749 w802 w849 w896 w943 w988 w1035 w1080 w1096 w1127 w1133 w1159 w1518 w1663 _ _]
      tunnel: w607 -> [w615 w622 w704 w740 w791 w838 w885 w932 w979 w1026 w1075 w1086 w1126 w1132 w1140 w1513 w1662 w1693 _]
      tunnel: [w615 w621 w703 w738 w790 w837 w884 w931 w978 w1025 w1074 w1085 w1124 w1130 w1148 w1512 w1662 w1693 _] -> w606
      tunnel: w605 -> [_ _ _ _ _ _ _ _ _ _ _ _ _ _ w1158 w1517 _ _ _]
      tunnel: [w614 w618 w699 w733 w781 w828 w875 w922 w969 w1016 w1063 w1082 w1123 w1129 w1147 w1511 w1665 w1687 _] -> w604
      tunnel: w603 -> [w614 w618 w699 w733 w781 w828 w875 w922 w969 w1016 w1063 w1082 w1123 w1129 w1147 w1511 w1665 w1688 _]
      tunnel: FALSE -> [_ w617 w698 w732 w780 w827 w874 w921 w968 w1015 w1062 w1081 w1122 w1128 w1146 w1510 _ w1686 _]
      tunnel: [TRUE w617 w698 w732 w780 w827 w874 w921 w968 w1015 w1062 w1081 w1122 w1128 w1146 w1510 TRUE w1686 _] -> w600
      tunnel: w599 -> [_ _ _ _ _ _ _ _ _ _ _ _ _ _ _ _ _ w1666 _]
      tunnel: w598 -> [_ _ _ _ _ _ _ _ _ _ _ _ _ _ _ _ _ w1667 _]
      event Timeout {
        n220 = event-data() -> ()  [unwired: 1 in, 3 out]
        n221 = property on="Save" class="Bool (strict)"("Val(Sgnl)"=TRUE) -> ()  [unwired: 2 in, 2 out]
      }
      event "Sample Type": Value Change {
        n222 = event-data() -> ("OldVal"=w624:u16, "CtlRef"=w629:refnum<vi>)  [unwired: 1 in]
        n223 = property class="Ring (strict)"(reference=w629) -> (reference out=w626:refnum<vi>, "Label.Text"=w623:string, "RingText.Text"=w620:string, "Value"=w619:u16)  [unwired: 1 in, 1 out]
        n224 = control-ref of="Sample Type Sub Types"() -> (w616:refnum<vi>)
        n225 = Equal?(x=w620, y="Add Item") -> (x = y?=w627:bool)
        n226 = case shown="False" w627 {
          tunnel: w626 -> [_ w657]
          tunnel: w625 -> [w641 w650]
          tunnel: w624 -> [_ w658]
          tunnel: w623 -> [_ w656]
          tunnel: w620 -> [w635 _]
          tunnel: w622 -> [w637 w655]
          tunnel: [w636 w654] -> w621
          tunnel: w619 -> [w634 _]
          tunnel: w616 -> [w631 w644]
          frame False {
            n227 = call "Populate Sub Menu.vi"("Sample Type Sub Types"=w631, "Base Path"=w641, "Ring Text"=w635) -> ("Sample Type Sub Types (Dup)"=w640:refnum<vi>, "Caption Text"=w639:string, "Menu Items"=w638:string[])  [unwired: 10 in]
            n228 = Bundle(cluster=T2 {"String"="", "Value"=0} ("Name Value Pair"), "String"=w635, "Value"=w634) -> (w633:T2)
            n229 = property class="Ring (strict)"(reference=w640, "Caption.Text"=w639, "Value"=u16 0, "Strings []"=w638) -> ()  [unwired: 1 in, 2 out]
            n230 = Bundle By Name(cluster=w637, "Sample Type"=w633) -> (w636:T1)
          }
          frame True {
            n231 = call "Add New Menu Item.vi"("Base Path"=w650, "Old Value"=w658, "Ring Menu Ref"=w657, "Label or Caption"=w656) -> ("New Item"=w643:string, "Menu Value"=w653:u16)  [unwired: 8 in, 2 out]
            n232 = Concatenate Strings("Enter " ("string"), w643, " Sub Type Name") -> (w649:string)
            n233 = call "Get User Input.vi"("Dialog Message"=w649) -> ("User Input"=w646:string, "Canceled?"=w647:bool)  [unwired: 13 in]
            n234 = case shown="False" w647 {
              tunnel: w650 -> [w683 _]
              tunnel: w646 -> [w677 _]
              tunnel: w644 -> [w684 _]
              tunnel: w643 -> [w671 _]
              frame False {
                w666 = string[][] []
                w678 = string[] ["Not Applicable", "-", "Add Item"]
                n235 = Build Array(w671, w677) -> (w676:string[])
                n236 = property class="Ring (strict)"(reference=w684, "Value"=u16 0, "Caption.Text"=w677, "Strings []"=w678) -> ("Label.Text"=w680:string)  [unwired: 1 in, 2 out]
                n237 = Concatenate Strings(w680, ".json" ("string")) -> (w681:string)
                n238 = Build Path(base path=w683, name or relative path=w680) -> (appended path=w661:path)
                n239 = Build Path(base path=w683, name or relative path=w681) -> (appended path=w672:path)
                n240 = call <vilib>:"Check if File or Folder Exists.vi"("path"=w661) -> ("error out"=w664:errorcluster, "file or folder exists?"=w662:bool, "dup path"=w663:path)  [unwired: 8 in]
                n241 = Read from Text File(file (use dialog)=w672) -> (text=w679:string, error out=w674:errorcluster)  [unwired: 3 in, 2 out]
                n242 = case shown="False" w662 {
                  tunnel: w663 -> [w693 w695]
                  tunnel: [w692 w695] -> w660
                  tunnel: w664 -> [w691 w694]
                  tunnel: [w690 w694] -> w659
                  frame False {
                    n243 = Create Folder(path (use dialog)=w693, error in=w691) -> (created path=w692:path, error out=w690:errorcluster)  [unwired: 1 in, 1 out]
                  }
                  frame True {
                  }
                }
                n244 = Unflatten From JSON(JSON string=w679, type and defaults=w666, error in (no error)=w674) -> (value=w668:string[][], error out=w669:errorcluster)  [unwired: 4 in]
                n245 = Concatenate Strings(w677, ".json" ("string")) -> (w688:string)
                n246 = case shown="No Error" w669 {
                  tunnel: [w696 w697] -> w667
                  tunnel: w668 -> [w696 _]
                  tunnel: w666 -> [_ w697]
                  frame No Error {
                  }
                  frame Error {
                  }
                }
                n247 = Build Path(base path=w660, name or relative path=w688) -> (appended path=w687:path)
                n248 = Flatten To JSON(anything=w678, error in (no error)=w659) -> (JSON string=w686:string, 11:w685:errorcluster)  [unwired: 1 in]
                n249 = Build Array (concatenate)(w667, w676) -> (w675:string[][])
                n250 = Flatten To JSON(anything=w675) -> (JSON string=w673:string, 11:w670:errorcluster)  [unwired: 2 in]
                n251 = Write to Text File(file (use dialog)=w687, text=w686, error in=w685) -> ()  [unwired: 1 in, 3 out]
                n252 = Write to Text File(file (use dialog)=w672, text=w673, error in=w670) -> ()  [unwired: 1 in, 3 out]
              }
              frame True {
              }
            }
            n253 = Bundle(cluster=T2 {"String"="", "Value"=0} ("Name Value Pair"), "String"=w643, "Value"=w653) -> (w652:T2)
            n254 = Bundle By Name(cluster=w655, "Sample Type"=w652) -> (w654:T1)
          }
        }
      }
      event "Sample Type Sub Types": Value Change {
        n255 = event-data() -> ("OldVal"=w707:u16, "CtlRef"=w711:refnum<vi>)  [unwired: 1 in]
        n256 = property class="Ring (strict)"(reference=w711) -> (reference out=w709:refnum<vi>, "Label.Text"=w705:string, "Caption.Text"=w706:string, "RingText.Text"=w702:string, "Value"=w701:u16)  [unwired: 1 in, 1 out]
        n257 = Equal?(x=w702, y="Add Item") -> (x = y?=w710:bool)
        n258 = case shown="True" w710 {
          tunnel: w709 -> [_ w731]
          tunnel: w708 -> [_ w729]
          tunnel: w707 -> [_ w730]
          tunnel: w706 -> [_ w728]
          tunnel: w705 -> [_ w727]
          tunnel: w704 -> [w719 w725]
          tunnel: [w718 w724] -> w703
          tunnel: w702 -> [w717 _]
          tunnel: w701 -> [w716 _]
          tunnel: T2 {"String"="", "Value"=0} ("Name Value Pair") -> [w714 w720]
          frame False {
            n259 = Bundle(cluster=w714, "String"=w717, "Value"=w716) -> (w715:T2)
            n260 = Bundle By Name(cluster=w719, "Sample Sub Type"=w715) -> (w718:T1)
          }
          frame True {
            n261 = Build Path(base path=w729, name or relative path=w727) -> (appended path=w726:path)
            n262 = call "Add New Menu Item.vi"("Base Path"=w726, "Old Value"=w730, "Ring Menu Ref"=w731, "Label or Caption"=w728) -> ("New Item"=w723:string, "Menu Value"=w722:u16)  [unwired: 8 in, 2 out]
            n263 = Bundle(cluster=w720, "String"=w723, "Value"=w722) -> (w721:T2)
            n264 = Bundle By Name(cluster=w725, "Sample Sub Type"=w721) -> (w724:T1)
          }
        }
      }
      event "Probe 1", "Probe 2", "Probe 3", "Probe 4": Value Change {
        n265 = event-data() -> ("CtlRef"=w748:refnum<vi>, "NewVal"=w737:bool)  [unwired: 1 in]
        n266 = property class="Bool (strict)"(reference=w748) -> ("Label.Text"=w747:string)  [unwired: 1 in, 2 out]
        n267 = Select(t=T6."Enabled" ("Disabled"), s=w737, f=T6."Disabled and Grayed Out" ("Disabled")) -> (s? t:f=w734:T6)
        n268 = case shown="\"Probe 2\"" w747 {
          tunnel: [w755 w762 w769 w776] -> w744
          tunnel: [0 1 2 3] -> w736
          tunnel: [w753 w760 w767 w774] -> w735
          frame "Probe 1", Default {
            n269 = control-ref of="Probe Name 01"() -> (w758:refnum<vi>)
            n270 = control-ref of="Probe Sub Type 01"() -> (w757:refnum<vi>)
            n271 = control-ref of="Probe Cat Num 01"() -> (w756:refnum<vi>)
            n272 = control-ref of="Probe Concentration 01"() -> (w753:refnum<vi>)
            n273 = control-ref of="Image Target 01"() -> (w752:refnum<vi>)
            n274 = Build Array(w758, w757, w756, w752) -> (w755:refnum<vi>[])
          }
          frame "Probe 2" {
            n275 = control-ref of="Probe Name 02"() -> (w765:refnum<vi>)
            n276 = control-ref of="Probe Sub Type 02"() -> (w764:refnum<vi>)
            n277 = control-ref of="Probe Cat Num 02"() -> (w763:refnum<vi>)
            n278 = control-ref of="Probe Concentration 02"() -> (w760:refnum<vi>)
            n279 = control-ref of="Image Target 02"() -> (w759:refnum<vi>)
            n280 = Build Array(w765, w764, w763, w759) -> (w762:refnum<vi>[])
          }
          frame "Probe 3" {
            n281 = control-ref of="Probe Name 03"() -> (w772:refnum<vi>)
            n282 = control-ref of="Probe Sub Type 03"() -> (w771:refnum<vi>)
            n283 = control-ref of="Probe Cat Num 03"() -> (w770:refnum<vi>)
            n284 = control-ref of="Probe Concentration 03"() -> (w767:refnum<vi>)
            n285 = control-ref of="Image Target 03"() -> (w766:refnum<vi>)
            n286 = Build Array(w772, w771, w770, w766) -> (w769:refnum<vi>[])
          }
          frame "Probe 4" {
            n287 = control-ref of="Probe Name 04"() -> (w779:refnum<vi>)
            n288 = control-ref of="Probe Sub Type 04"() -> (w778:refnum<vi>)
            n289 = control-ref of="Probe Cat Num 04"() -> (w777:refnum<vi>)
            n290 = control-ref of="Probe Concentration 04"() -> (w774:refnum<vi>)
            n291 = control-ref of="Image Target 04"() -> (w773:refnum<vi>)
            n292 = Build Array(w779, w778, w777, w773) -> (w776:refnum<vi>[])
          }
        }
        n293 = property class="DigNum (strict)"(reference=w735, "DisabledEnum"=w734) -> ()  [unwired: 1 in, 2 out]
        n294 = for {
          tunnel: w744 -> [w751] mode=indexing
          tunnel: w734 -> [w750]
          n295 = property class="Ring (strict)"(reference=w751, "DisabledEnum"=w750) -> ()  [unwired: 1 in, 2 out]
        }
        n296 = Unbundle By Name(w740) -> ("Proble Data"=w742:T3[])
        n297 = Index Array(array=w742, index=w736) -> (element=w743:T3)
        n298 = Bundle By Name(cluster=w743, "Active?"=w737) -> (w741:T3)
        n299 = Replace Array Subset(array=w742, new element=w741, index=w736) -> (w739:T3[])
        n300 = Bundle By Name(cluster=w740, "Proble Data"=w739) -> (w738:T1)
      }
      event "Probe Name 01", "Probe Name 02", "Probe Name 03", "Probe Name 04": Value Change {
        n301 = event-data() -> ("OldVal"=w797:u16, "CtlRef"=w796:refnum<vi>)  [unwired: 1 in]
        n302 = property class="Ring (strict)"(reference=w796) -> (reference out=w799:refnum<vi>, "Label.Text"=w784:string, "RingText.Text"=w787:string, "Value"=w786:u16)  [unwired: 1 in, 1 out]
        n303 = call "Get Label Text and Index.vi"("Label Text and Index"=w784) -> ("Text"=w782:string, "Index"=w783:i32)  [unwired: 12 in, 1 out]
        n304 = Equal?(x=w787, y="Add Item") -> (x = y?=w800:bool)
        n305 = case shown="True" w800 {
          tunnel: w799 -> [_ w824]
          tunnel: w798 -> [_ w822]
          tunnel: w797 -> [_ w823]
          tunnel: [w803 w809] -> w789
          tunnel: [w804 w811] -> w788
          tunnel: w787 -> [w806 _]
          tunnel: w786 -> [w805 _]
          tunnel: T2 {"String"="", "Value"=0} ("Name Value Pair") -> [w807 w810]
          tunnel: w782 -> [_ w808]
          tunnel: w783 -> [w803 w809]
          frame False {
            n306 = Bundle(cluster=w807, "String"=w806, "Value"=w805) -> (w804:T2)
          }
          frame True {
            n307 = control-ref of="Probe Name 01"() -> (w817:refnum<vi>)
            n308 = control-ref of="Probe Name 02"() -> (w820:refnum<vi>)
            n309 = control-ref of="Probe Name 03"() -> (w819:refnum<vi>)
            n310 = control-ref of="Probe Name 04"() -> (w818:refnum<vi>)
            n311 = call "Add New Menu Item.vi"("Base Path"=w822, "Old Value"=w823, "Ring Menu Ref"=w824, "Label or Caption"=w808) -> ("Menu Strings"=w821:string[], "New Item"=w812:string, "Menu Value"=w813:u16)  [unwired: 8 in, 1 out]
            n312 = Bundle(cluster=w810, "String"=w812, "Value"=w813) -> (w811:T2)
            n313 = Build Array(w817, w820, w819, w818) -> (w816:refnum<vi>[])
            n314 = Delete From Array(array=w816, length=1, index=w809) -> (array with subset deleted=w814:refnum<vi>[])  [unwired: 1 out]
            n315 = for {
              tunnel: w814 -> [w826] mode=indexing
              tunnel: w821 -> [w825]
              n316 = property class="Ring (strict)"(reference=w826, "Strings []"=w825) -> ()  [unwired: 1 in, 2 out]
            }
          }
        }
        n317 = Unbundle By Name(w791) -> ("Proble Data"=w794:T3[])
        n318 = Index Array(array=w794, index=w789) -> (element=w795:T3)
        n319 = Bundle By Name(cluster=w795, "Name"=w788) -> (w793:T3)
        n320 = Replace Array Subset(array=w794, new element=w793, index=w789) -> (w792:T3[])
        n321 = Bundle By Name(cluster=w791, "Proble Data"=w792) -> (w790:T1)
      }
      event "Image Target 01", "Image Target 02", "Image Target 03", "Image Target 04": Value Change {
        n322 = event-data() -> ("OldVal"=w844:u16, "CtlRef"=w843:refnum<vi>)  [unwired: 1 in]
        n323 = property class="Ring (strict)"(reference=w843) -> (reference out=w846:refnum<vi>, "Label.Text"=w831:string, "RingText.Text"=w834:string, "Value"=w833:u16)  [unwired: 1 in, 1 out]
        n324 = call "Get Label Text and Index.vi"("Label Text and Index"=w831) -> ("Text"=w829:string, "Index"=w830:i32)  [unwired: 12 in, 1 out]
        n325 = Equal?(x=w834, y="Add Item") -> (x = y?=w847:bool)
        n326 = case shown="True" w847 {
          tunnel: w846 -> [_ w871]
          tunnel: w845 -> [_ w869]
          tunnel: w844 -> [_ w870]
          tunnel: [w850 w855] -> w836
          tunnel: [w851 w858] -> w835
          tunnel: w834 -> [w853 _]
          tunnel: w833 -> [w852 _]
          tunnel: T2 {"String"="", "Value"=0} ("Name Value Pair") -> [w854 w857]
          tunnel: w829 -> [_ w856]
          tunnel: w830 -> [w850 w855]
          frame False {
            n327 = Bundle(cluster=w854, "String"=w853, "Value"=w852) -> (w851:T2)
          }
          frame True {
            n328 = control-ref of="Image Target 01"() -> (w864:refnum<vi>)
            n329 = control-ref of="Image Target 02"() -> (w867:refnum<vi>)
            n330 = control-ref of="Image Target 03"() -> (w866:refnum<vi>)
            n331 = control-ref of="Image Target 04"() -> (w865:refnum<vi>)
            n332 = call "Add New Menu Item.vi"("Base Path"=w869, "Old Value"=w870, "Ring Menu Ref"=w871, "Label or Caption"=w856) -> ("Menu Strings"=w868:string[], "New Item"=w859:string, "Menu Value"=w860:u16)  [unwired: 8 in, 1 out]
            n333 = Bundle(cluster=w857, "String"=w859, "Value"=w860) -> (w858:T2)
            n334 = Build Array(w864, w867, w866, w865) -> (w863:refnum<vi>[])
            n335 = Delete From Array(array=w863, length=1, index=w855) -> (array with subset deleted=w861:refnum<vi>[])  [unwired: 1 out]
            n336 = for {
              tunnel: w861 -> [w873] mode=indexing
              tunnel: w868 -> [w872]
              n337 = property class="Ring (strict)"(reference=w873, "Strings []"=w872) -> ()  [unwired: 1 in, 2 out]
            }
          }
        }
        n338 = Unbundle By Name(w838) -> ("Proble Data"=w841:T3[])
        n339 = Index Array(array=w841, index=w836) -> (element=w842:T3)
        n340 = Bundle By Name(cluster=w842, "Target"=w835) -> (w840:T3)
        n341 = Replace Array Subset(array=w841, new element=w840, index=w836) -> (w839:T3[])
        n342 = Bundle By Name(cluster=w838, "Proble Data"=w839) -> (w837:T1)
      }
      event "Probe Sub Type 01", "Probe Sub Type 02", "Probe Sub Type 03", "Probe Sub Type 04": Value Change {
        n343 = event-data() -> ("OldVal"=w891:u16, "CtlRef"=w890:refnum<vi>)  [unwired: 1 in]
        n344 = property class="Ring (strict)"(reference=w890) -> (reference out=w893:refnum<vi>, "Label.Text"=w878:string, "RingText.Text"=w881:string, "Value"=w880:u16)  [unwired: 1 in, 1 out]
        n345 = call "Get Label Text and Index.vi"("Label Text and Index"=w878) -> ("Text"=w876:string, "Index"=w877:i32)  [unwired: 12 in, 1 out]
        n346 = Equal?(x=w881, y="Add Item") -> (x = y?=w894:bool)
        n347 = case shown="True" w894 {
          tunnel: w893 -> [_ w918]
          tunnel: w892 -> [_ w915]
          tunnel: w891 -> [_ w917]
          tunnel: w876 -> [_ w916]
          tunnel: [w897 w902] -> w883
          tunnel: [w898 w904] -> w882
          tunnel: w881 -> [w900 _]
          tunnel: w880 -> [w899 _]
          tunnel: T2 {"String"="", "Value"=0} ("Name Value Pair") -> [w901 w903]
          tunnel: w877 -> [w897 w902]
          frame False {
            n348 = Bundle(cluster=w901, "String"=w900, "Value"=w899) -> (w898:T2)
          }
          frame True {
            n349 = control-ref of="Probe Sub Type 01"() -> (w910:refnum<vi>)
            n350 = control-ref of="Probe Sub Type 02"() -> (w913:refnum<vi>)
            n351 = control-ref of="Probe Sub Type 03"() -> (w912:refnum<vi>)
            n352 = control-ref of="Probe Sub Type 04"() -> (w911:refnum<vi>)
            n353 = call "Add New Menu Item.vi"("Base Path"=w915, "Old Value"=w917, "Ring Menu Ref"=w918, "Label or Caption"=w916) -> ("Menu Strings"=w914:string[], "New Item"=w905:string, "Menu Value"=w906:u16)  [unwired: 8 in, 1 out]
            n354 = Bundle(cluster=w903, "String"=w905, "Value"=w906) -> (w904:T2)
            n355 = Build Array(w910, w913, w912, w911) -> (w909:refnum<vi>[])
            n356 = Delete From Array(array=w909, length=1, index=w902) -> (array with subset deleted=w907:refnum<vi>[])  [unwired: 1 out]
            n357 = for {
              tunnel: w907 -> [w920] mode=indexing
              tunnel: w914 -> [w919]
              n358 = property class="Ring (strict)"(reference=w920, "Strings []"=w919) -> ()  [unwired: 1 in, 2 out]
            }
          }
        }
        n359 = Unbundle By Name(w885) -> ("Proble Data"=w888:T3[])
        n360 = Index Array(array=w888, index=w883) -> (element=w889:T3)
        n361 = Bundle By Name(cluster=w889, "Sub Type"=w882) -> (w887:T3)
        n362 = Replace Array Subset(array=w888, new element=w887, index=w883) -> (w886:T3[])
        n363 = Bundle By Name(cluster=w885, "Proble Data"=w886) -> (w884:T1)
      }
      event "Probe Cat Num 01", "Probe Cat Num 02", "Probe Cat Num 03", "Probe Cat Num 04": Value Change {
        n364 = event-data() -> ("OldVal"=w938:u16, "CtlRef"=w937:refnum<vi>)  [unwired: 1 in]
        n365 = property class="Ring (strict)"(reference=w937) -> (reference out=w940:refnum<vi>, "Label.Text"=w926:string, "RingText.Text"=w925:string, "Value"=w928:u16)  [unwired: 1 in, 1 out]
        n366 = call "Get Label Text and Index.vi"("Label Text and Index"=w926) -> ("Text"=w923:string, "Index"=w924:i32)  [unwired: 12 in, 1 out]
        n367 = Equal?(x=w925, y="Add Item") -> (x = y?=w941:bool)
        n368 = case shown="True" w941 {
          tunnel: w940 -> [_ w965]
          tunnel: w939 -> [_ w963]
          tunnel: w938 -> [_ w964]
          tunnel: [w944 w949] -> w930
          tunnel: [w946 w952] -> w929
          tunnel: w928 -> [w947 _]
          tunnel: T2 {"String"="", "Value"=0} ("Name Value Pair") -> [w948 w951]
          tunnel: w923 -> [_ w950]
          tunnel: w925 -> [w945 _]
          tunnel: w924 -> [w944 w949]
          frame False {
            n369 = Bundle(cluster=w948, "String"=w945, "Value"=w947) -> (w946:T2)
          }
          frame True {
            n370 = control-ref of="Probe Cat Num 01"() -> (w958:refnum<vi>)
            n371 = control-ref of="Probe Cat Num 02"() -> (w961:refnum<vi>)
            n372 = control-ref of="Probe Cat Num 03"() -> (w960:refnum<vi>)
            n373 = control-ref of="Probe Cat Num 04"() -> (w959:refnum<vi>)
            n374 = call "Add New Menu Item.vi"("Base Path"=w963, "Old Value"=w964, "Ring Menu Ref"=w965, "Label or Caption"=w950) -> ("Menu Strings"=w962:string[], "New Item"=w953:string, "Menu Value"=w954:u16)  [unwired: 8 in, 1 out]
            n375 = Bundle(cluster=w951, "String"=w953, "Value"=w954) -> (w952:T2)
            n376 = Build Array(w958, w961, w960, w959) -> (w957:refnum<vi>[])
            n377 = Delete From Array(array=w957, length=1, index=w949) -> (array with subset deleted=w955:refnum<vi>[])  [unwired: 1 out]
            n378 = for {
              tunnel: w955 -> [w967] mode=indexing
              tunnel: w962 -> [w966]
              n379 = property class="Ring (strict)"(reference=w967, "Strings []"=w966) -> ()  [unwired: 1 in, 2 out]
            }
          }
        }
        n380 = Unbundle By Name(w932) -> ("Proble Data"=w935:T3[])
        n381 = Index Array(array=w935, index=w930) -> (element=w936:T3)
        n382 = Bundle By Name(cluster=w936, "Cat Number"=w929) -> (w934:T3)
        n383 = Replace Array Subset(array=w935, new element=w934, index=w930) -> (w933:T3[])
        n384 = Bundle By Name(cluster=w932, "Proble Data"=w933) -> (w931:T1)
      }
      event "Extra Tag 01", "Extra Tag 02", "Extra Tag 03", "Extra Tag 04", "Extra Tag 05", "Extra Tag 06": Value Change {
        n385 = event-data() -> ("OldVal"=w983:u16, "CtlRef"=w982:refnum<vi>)  [unwired: 1 in]
        n386 = property class="Ring (strict)"(reference=w982) -> (reference out=w985:refnum<vi>, "Label.Text"=w972:string, "RingText.Text"=w977:string, "Value"=w976:u16)  [unwired: 1 in, 1 out]
        n387 = call "Get Label Text and Index.vi"("Label Text and Index"=w972) -> ("Text"=w970:string, "Index"=w971:i32)  [unwired: 12 in, 1 out]
        n388 = Equal?(x=w977, y="Add Item") -> (x = y?=w986:bool)
        n389 = case shown="False" w986 {
          tunnel: w985 -> [_ w1012]
          tunnel: w984 -> [_ w1009]
          tunnel: w983 -> [_ w1011]
          tunnel: w970 -> [_ w1010]
          tunnel: [w989 w994] -> w974
          tunnel: [w990 w998] -> w973
          tunnel: w977 -> [w992 _]
          tunnel: w976 -> [w991 _]
          tunnel: T2 {"String"="", "Value"=0} ("Name Value Pair") -> [w993 w997]
          tunnel: w971 -> [w989 w994]
          frame False {
            n390 = Bundle(cluster=w993, "String"=w992, "Value"=w991) -> (w990:T2)
          }
          frame True {
            n391 = control-ref of="Extra Tag 01"() -> (w1004:refnum<vi>)
            n392 = control-ref of="Extra Tag 02"() -> (w1007:refnum<vi>)
            n393 = control-ref of="Extra Tag 03"() -> (w1006:refnum<vi>)
            n394 = control-ref of="Extra Tag 04"() -> (w1005:refnum<vi>)
            n395 = control-ref of="Extra Tag 05"() -> (w996:refnum<vi>)
            n396 = control-ref of="Extra Tag 06"() -> (w995:refnum<vi>)
            n397 = call "Add New Menu Item.vi"("Base Path"=w1009, "Old Value"=w1011, "Ring Menu Ref"=w1012, "Label or Caption"=w1010) -> ("Menu Strings"=w1008:string[], "New Item"=w999:string, "Menu Value"=w1000:u16)  [unwired: 8 in, 1 out]
            n398 = Bundle(cluster=w997, "String"=w999, "Value"=w1000) -> (w998:T2)
            n399 = Build Array(w1004, w1007, w1006, w1005, w996, w995) -> (w1003:refnum<vi>[])
            n400 = Delete From Array(array=w1003, length=1, index=w994) -> (array with subset deleted=w1001:refnum<vi>[])  [unwired: 1 out]
            n401 = for {
              tunnel: w1001 -> [w1014] mode=indexing
              tunnel: w1008 -> [w1013]
              n402 = property class="Ring (strict)"(reference=w1014, "Strings []"=w1013) -> ()  [unwired: 1 in, 2 out]
            }
          }
        }
        n403 = Unbundle By Name(w979) -> ("Extra Tags"=w981:T2[])
        n404 = Replace Array Subset(array=w981, new element=w973, index=w974) -> (w980:T2[])
        n405 = Bundle By Name(cluster=w979, "Extra Tags"=w980) -> (w978:T1)
      }
      event "Scavenger 01", "Scavenger 02", "Scavenger 03", "Scavenger 04", "Scavenger 05", "Scavenger 06": Value Change {
        n406 = event-data() -> ("OldVal"=w1030:u16, "CtlRef"=w1029:refnum<vi>)  [unwired: 1 in]
        n407 = property class="Ring (strict)"(reference=w1029) -> (reference out=w1032:refnum<vi>, "Label.Text"=w1019:string, "RingText.Text"=w1024:string, "Value"=w1023:u16)  [unwired: 1 in, 1 out]
        n408 = call "Get Label Text and Index.vi"("Label Text and Index"=w1019) -> ("Text"=w1017:string, "Index"=w1018:i32)  [unwired: 12 in, 1 out]
        n409 = Equal?(x=w1024, y="Add Item") -> (x = y?=w1033:bool)
        n410 = case shown="True" w1033 {
          tunnel: w1032 -> [_ w1059]
          tunnel: w1031 -> [_ w1056]
          tunnel: w1030 -> [_ w1058]
          tunnel: w1017 -> [_ w1057]
          tunnel: [w1036 w1041] -> w1021
          tunnel: [w1037 w1045] -> w1020
          tunnel: w1024 -> [w1039 _]
          tunnel: w1023 -> [w1038 _]
          tunnel: T2 {"String"="", "Value"=0} ("Name Value Pair") -> [w1040 w1044]
          tunnel: w1018 -> [w1036 w1041]
          frame False {
            n411 = Bundle(cluster=w1040, "String"=w1039, "Value"=w1038) -> (w1037:T2)
          }
          frame True {
            n412 = control-ref of="Scavenger 01"() -> (w1051:refnum<vi>)
            n413 = control-ref of="Scavenger 02"() -> (w1054:refnum<vi>)
            n414 = control-ref of="Scavenger 03"() -> (w1053:refnum<vi>)
            n415 = control-ref of="Scavenger 04"() -> (w1052:refnum<vi>)
            n416 = control-ref of="Scavenger 05"() -> (w1043:refnum<vi>)
            n417 = control-ref of="Scavenger 06"() -> (w1042:refnum<vi>)
            n418 = call "Add New Menu Item.vi"("Base Path"=w1056, "Old Value"=w1058, "Ring Menu Ref"=w1059, "Label or Caption"=w1057) -> ("Menu Strings"=w1055:string[], "New Item"=w1046:string, "Menu Value"=w1047:u16)  [unwired: 8 in, 1 out]
            n419 = Bundle(cluster=w1044, "String"=w1046, "Value"=w1047) -> (w1045:T2)
            n420 = Build Array(w1051, w1054, w1053, w1052, w1043, w1042) -> (w1050:refnum<vi>[])
            n421 = Delete From Array(array=w1050, length=1, index=w1041) -> (array with subset deleted=w1048:refnum<vi>[])  [unwired: 1 out]
            n422 = for {
              tunnel: w1048 -> [w1061] mode=indexing
              tunnel: w1055 -> [w1060]
              n423 = property class="Ring (strict)"(reference=w1061, "Strings []"=w1060) -> ()  [unwired: 1 in, 2 out]
            }
          }
        }
        n424 = Unbundle By Name(w1026) -> ("Scavenger Tags"=w1028:T2[])
        n425 = Replace Array Subset(array=w1028, new element=w1020, index=w1021) -> (w1027:T2[])
        n426 = Bundle By Name(cluster=w1026, "Scavenger Tags"=w1027) -> (w1025:T1)
      }
      event "Probe Concentration 01", "Probe Concentration 02", "Probe Concentration 03", "Probe Concentration 04": Value Change {
        n427 = event-data() -> ("CtlRef"=w1067:refnum<vi>, "NewVal"=w1064:dbl)  [unwired: 1 in]
        n428 = property class="DigNum (strict)"(reference=w1067) -> ("Label.Text"=w1066:string)  [unwired: 1 in, 2 out]
        n429 = String Length(string=w1066) -> (length=w1073:i32)
        n430 = Subtract(x=w1073, y=2) -> (x-y=w1071:i32)
        n431 = To Unsigned Long Integer(number=w1071) -> (unsigned 32bit integer=w1070:u32)
        n432 = Unbundle By Name(w1075) -> ("Proble Data"=w1078:T3[])
        n433 = Scan From String(input string=w1066, initial scan location=w1070, default 1=0 ("y")) -> (output 1=w1068:i32)  [unwired: 2 in, 3 out]
        n434 = Decrement(x=w1068) -> (x-1=w1065:i32)
        n435 = Index Array(array=w1078, index=w1065) -> (element=w1079:T3)
        n436 = Bundle By Name(cluster=w1079, "Concentration"=w1064) -> (w1077:T3)
        n437 = Replace Array Subset(array=w1078, new element=w1077, index=w1065) -> (w1076:T3[])
        n438 = Bundle By Name(cluster=w1075, "Proble Data"=w1076) -> (w1074:T1)
      }
      event "Buffer Type", "Sample Holder", "Sealant", "User Name": Value Change {
        n439 = event-data() -> ("OldVal"=w1090:u16, "CtlRef"=w1091:refnum<vi>)  [unwired: 1 in]
        n440 = property class="Ring (strict)"(reference=w1091) -> (reference out=w1093:refnum<vi>, "Label.Text"=w1084:string, "RingText.Text"=w1088:string, "Value"=w1092:u16)  [unwired: 1 in, 1 out]
        n441 = Equal?(x=w1088, y="Add Item") -> (x = y?=w1094:bool)
        n442 = case shown="False" w1094 {
          tunnel: w1093 -> [_ w1119]
          tunnel: w1089 -> [_ w1121]
          tunnel: w1090 -> [_ w1120]
          tunnel: w1084 -> [_ w1118]
          tunnel: w1088 -> [w1113 _]
          tunnel: w1092 -> [w1112 _]
          tunnel: [w1111 w1115] -> w1087
          tunnel: T2 {"String"="", "Value"=0} ("Name Value Pair") -> [w1110 w1114]
          frame False {
            n443 = Bundle(cluster=w1110, "String"=w1113, "Value"=w1112) -> (w1111:T2)
          }
          frame True {
            n444 = call "Add New Menu Item.vi"("Base Path"=w1121, "Old Value"=w1120, "Ring Menu Ref"=w1119, "Label or Caption"=w1118) -> ("New Item"=w1117:string, "Menu Value"=w1116:u16)  [unwired: 8 in, 2 out]
            n445 = Bundle(cluster=w1114, "String"=w1117, "Value"=w1116) -> (w1115:T2)
          }
        }
        n446 = case shown="\"Sample Holder\"" w1084 {
          tunnel: w1087 -> [_ w1099 w1103 w1106 w1109]
          tunnel: w1086 -> [w1097 w1100 w1102 w1105 w1108]
          tunnel: [w1097 w1098 w1101 w1104 w1107] -> w1085
          frame Default {
          }
          frame "Buffer Type" {
            n447 = Bundle By Name(cluster=w1100, "Buffer Type"=w1099) -> (w1098:T1)
          }
          frame "Sample Holder" {
            n448 = Bundle By Name(cluster=w1102, "Sample Holder"=w1103) -> (w1101:T1)
          }
          frame "Sealant" {
            n449 = Bundle By Name(cluster=w1105, "Sealant"=w1106) -> (w1104:T1)
          }
          frame "User Name" {
            n450 = Bundle By Name(cluster=w1108, "User Name"=w1109) -> (w1107:T1)
          }
        }
      }
      event "Buffer PH": Value Change {
        n451 = event-data() -> ("NewVal"=w1125:dbl)  [unwired: 1 in]
        n452 = Bundle By Name(cluster=w1126, "Buffer PH"=w1125) -> (w1124:T1)
      }
      event "Notes": Value Change {
        n453 = event-data() -> ("NewVal"=w1131:string)  [unwired: 1 in]
        n454 = Bundle By Name(cluster=w1132, "Notes"=w1131) -> (w1130:T1)
      }
      event "Preset Metadata", "Load Preset": Value Change {
        n455 = event-data() -> ("CtlRef"=w1157:refnum<vi>)  [unwired: 1 in]
        n456 = property class="Ctl"(reference=w1157) -> (reference out=w1155:refnum<vi>, "Label.Text"=w1156:string)  [unwired: 1 in, 1 out]
        n457 = control-ref of="This VI"() -> (w1154:refnum<vi>)
        n458 = property class="VI"(reference=w1154) -> (error out=w1152:errorcluster, "Panel"=w1153:refnum<vi>)  [unwired: 1 in, 1 out]
        n459 = property class="Pnl"(reference=w1153, error in=w1152) -> (error out=w1151:errorcluster, "Controls[]"=w1150:refnum<vi>[])  [unwired: 1 out]
        n460 = case shown="\"Preset Metadata\"" w1156 {
          tunnel: w1158 -> [w1497 w1508]
          tunnel: w1155 -> [_ w1506]
          tunnel: w1151 -> [w1496 w1503]
          tunnel: [w1495 w1501] -> w1143
          tunnel: [w1494 w1500] -> w1142
          frame "Load Preset", Default {
            n461 = call "File Dialog"("start path"=w1497, "prompt"="Select Metadata File", "error in"=w1496, "pattern label"="*.json") -> ("selected path"=w1495:path, "error out"=w1494:errorcluster)  [unwired: 8 in, 2 out]
          }
          frame "Preset Metadata" {
            w1505 = refnum<vi> refnum  # Ring
            n462 = To More Specific Class(target class=w1505, reference=w1506) -> (specific class reference=w1504:refnum<vi>)  [unwired: 1 in, 1 out]
            n463 = property class="Ring"(reference=w1504, error in=w1503) -> (error out=w1500:errorcluster, "RingText.Text"=w1502:string)  [unwired: 1 out]
            n464 = Concatenate Strings(w1502, ".json" ("string")) -> (w1507:string)
            n465 = Build Path(base path=w1508, name or relative path=w1507) -> (appended path=w1501:path)
          }
        }
        n466 = Read from Text File(file (use dialog)=w1143, error in=w1142) -> (text=w1145:string, error out=w1144:errorcluster)  [unwired: 2 in, 2 out]
        n467 = Unflatten From JSON(JSON string=w1145, type and defaults=w1140, error in (no error)=w1144) -> (value=w1141:T1, error out=w1139:errorcluster)  [unwired: 4 in]
        n468 = Unbundle By Name(w1139) -> ("status"=w1136:bool, "code"=w1138:i32)
        n469 = Not Equal?(x=w1138, y=-375006) -> (x != y?=w1135:bool)
        n470 = And(x=w1136, y=w1135) -> (x .and. y?=w1134:bool)
        n471 = case shown="False" w1134 {
          tunnel: [w1160 w1493] -> w1148
          tunnel: w1150 -> [w1162 _]
          tunnel: w1149 -> [w1161 _]
          tunnel: w1140 -> [_ w1493]
          tunnel: w1141 -> [w1160 _]
          frame False {
            n472 = for {
              tunnel: w1162 -> [w1169] mode=indexing
              tunnel: w1160 -> [w1167]
              tunnel: w1161 -> [w1166]
              n473 = property class="Ctl"(reference=w1169) -> (reference out=w1168:refnum<vi>, "Label.Text"=w1165:string)  [unwired: 1 in, 1 out]
              n474 = call "Get Label Text and Index.vi"("Label Text and Index"=w1165) -> ("Label Text and Index (Dup)"=w1164:string, "Index"=w1163:i32)  [unwired: 12 in, 1 out]
              n475 = case shown="\"Buffer PH\"" w1164 {
                tunnel: w1168 -> [_ w1178 w1313 w1319 w1325 w1331 w1337 w1343 w1358 w1378 w1398 w1418 w1430 w1439 w1448 w1457 w1466 w1475 w1484 w1490]
                tunnel: w1167 -> [_ w1176 w1311 w1317 w1323 w1329 w1335 w1341 w1362 w1382 w1402 w1422 w1433 w1442 w1451 w1460 w1469 w1478 w1487 w1489]
                tunnel: w1166 -> [_ _ w1301 _ _ _ _ _ _ _ _ _ _ _ _ _ _ _ _ _]
                tunnel: w1163 -> [_ _ _ _ _ _ _ _ w1345 w1365 w1385 w1405 w1425 w1434 w1443 w1452 w1461 w1470 w1479 _]
                frame Default {
                }
                frame "Preset Metadata" {
                  w1179 = refnum<vi> refnum  # Ring
                  n476 = Unbundle By Name(w1176) -> ("Preset Name"=w1171:string)
                  n477 = To More Specific Class(target class=w1179, reference=w1178) -> (specific class reference=w1177:refnum<vi>)  [unwired: 1 in, 1 out]
                  n478 = control-ref of="Preset Metadata"() -> (w1173:refnum<vi>)
                  n479 = property class="Ring (strict)"(reference=w1173) -> ("Strings []"=w1174:string[])  [unwired: 1 in, 2 out]
                  n480 = for {
                    tunnel: w1171 -> [w1186]
                    tunnel: w1174 -> [w1184] mode=indexing
                    tunnel: [w1180] -> w1172
                    i -> [w1180]
                    stop <- w1183 stop-if-true
                    n481 = xnode "Match Regular Expression"("input string"=w1184, "regular expression"=w1186, "ignore case? (F)"=FALSE) -> ("whole match"=w1182:string)  [unwired: 3 in, 4 out]
                    n482 = Not Equal?(x=w1182, y="") -> (x != y?=w1183:bool)
                  }
                  n483 = To Unsigned Word Integer(number=w1172) -> (unsigned 16bit integer=w1170:u16)
                  n484 = To Variant(anything=w1170) -> (Variant=w1175:variant)
                  n485 = property class="Ring"(reference=w1177, "Value"=w1175) -> ()  [unwired: 1 in, 2 out]
                }
                frame "Sample Type" {
                  w1314 = refnum<vi> refnum  # Ring
                  n486 = Unbundle By Name(w1311) -> ("Sample Type.Value"=w1310:u16)
                  n487 = To More Specific Class(target class=w1314, reference=w1313) -> (specific class reference=w1312:refnum<vi>)  [unwired: 1 in, 1 out]
                  n488 = To Variant(anything=w1310) -> (Variant=w1309:variant)
                  n489 = property class="Ring"(reference=w1312, "Value"=w1309) -> (reference out=w1308:refnum<vi>)  [unwired: 1 in, 1 out]
                  n490 = property class="Ring"(reference=w1308) -> ("RingText.Text"=w1302:string)  [unwired: 1 in, 2 out]
                  n491 = control-ref of="Sample Type Sub Types"() -> (w1306:refnum<vi>)
                  n492 = call "Populate Sub Menu.vi"("Sample Type Sub Types"=w1306, "Base Path"=w1301, "Ring Text"=w1302) -> ("Sample Type Sub Types (Dup)"=w1305:refnum<vi>, "Caption Text"=w1304:string, "Menu Items"=w1303:string[])  [unwired: 10 in]
                  n493 = property class="Ring (strict)"(reference=w1305, "Caption.Text"=w1304, "Value"=u16 0, "Strings []"=w1303) -> ()  [unwired: 1 in, 2 out]
                }
                frame "Sample Type Sub Types" {
                  w1320 = refnum<vi> refnum  # Ring
                  n494 = Unbundle By Name(w1317) -> ("Sample Sub Type.Value"=w1316:u16)
                  n495 = To More Specific Class(target class=w1320, reference=w1319) -> (specific class reference=w1318:refnum<vi>)  [unwired: 1 in, 1 out]
                  n496 = To Variant(anything=w1316) -> (Variant=w1315:variant)
                  n497 = property class="Ring"(reference=w1318, "Value"=w1315) -> ()  [unwired: 1 in, 2 out]
                }
                frame "Sample Holder" {
                  w1326 = refnum<vi> refnum  # Ring
                  n498 = Unbundle By Name(w1323) -> ("Sample Holder.Value"=w1322:u16)
                  n499 = To More Specific Class(target class=w1326, reference=w1325) -> (specific class reference=w1324:refnum<vi>)  [unwired: 1 in, 1 out]
                  n500 = To Variant(anything=w1322) -> (Variant=w1321:variant)
                  n501 = property class="Ring"(reference=w1324, "Value"=w1321) -> ()  [unwired: 1 in, 2 out]
                }
                frame "Sealant" {
                  w1332 = refnum<vi> refnum  # Ring
                  n502 = Unbundle By Name(w1329) -> ("Sealant.Value"=w1328:u16)
                  n503 = To More Specific Class(target class=w1332, reference=w1331) -> (specific class reference=w1330:refnum<vi>)  [unwired: 1 in, 1 out]
                  n504 = To Variant(anything=w1328) -> (Variant=w1327:variant)
                  n505 = property class="Ring"(reference=w1330, "Value"=w1327) -> ()  [unwired: 1 in, 2 out]
                }
                frame "Buffer Type" {
                  w1338 = refnum<vi> refnum  # Ring
                  n506 = Unbundle By Name(w1335) -> ("Buffer Type.Value"=w1334:u16)
                  n507 = To More Specific Class(target class=w1338, reference=w1337) -> (specific class reference=w1336:refnum<vi>)  [unwired: 1 in, 1 out]
                  n508 = To Variant(anything=w1334) -> (Variant=w1333:variant)
                  n509 = property class="Ring"(reference=w1336, "Value"=w1333) -> ()  [unwired: 1 in, 2 out]
                }
                frame "Buffer PH" {
                  w1344 = refnum<vi> refnum  # Numeric
                  n510 = Unbundle By Name(w1341) -> ("Buffer PH"=w1340:dbl)
                  n511 = To More Specific Class(target class=w1344, reference=w1343) -> (specific class reference=w1342:refnum<vi>)  [unwired: 1 in, 1 out]
                  n512 = To Variant(anything=w1340) -> (Variant=w1339:variant)
                  n513 = property class="Num"(reference=w1342, "Value"=w1339) -> ()  [unwired: 1 in, 2 out]
                }
                frame "Probe 1" {
                  w1359 = refnum<vi> refnum  # Boolean
                  n514 = Unbundle By Name(w1362) -> ("Proble Data"=w1361:T3[])
                  n515 = To More Specific Class(target class=w1359, reference=w1358) -> (specific class reference=w1357:refnum<vi>)  [unwired: 1 in, 1 out]
                  n516 = Index Array(array=w1361, index=w1345) -> (element=w1360:T3)
                  n517 = Unbundle By Name(w1360) -> ("Active?"=w1347:bool)
                  n518 = To Variant(anything=w1347) -> (Variant=w1356:variant)
                  n519 = Select(t=T6."Enabled" ("Disabled"), s=w1347, f=T6."Disabled and Grayed Out" ("Disabled")) -> (s? t:f=w1346:T6)
                  n520 = property class="Bool"(reference=w1357, "Value"=w1356) -> ()  [unwired: 1 in, 2 out]
                  n521 = control-ref of="Probe Name 01"() -> (w1352:refnum<vi>)
                  n522 = control-ref of="Image Target 01"() -> (w1353:refnum<vi>)
                  n523 = control-ref of="Probe Sub Type 01"() -> (w1354:refnum<vi>)
                  n524 = control-ref of="Probe Cat Num 01"() -> (w1355:refnum<vi>)
                  n525 = control-ref of="Probe Concentration 01"() -> (w1350:refnum<vi>)
                  n526 = Build Array(w1352, w1353, w1354, w1355) -> (w1351:refnum<vi>[])
                  n527 = for {
                    tunnel: w1351 -> [w1364] mode=indexing
                    tunnel: w1346 -> [w1363]
                    n528 = property class="Ring (strict)"(reference=w1364, "DisabledEnum"=w1363) -> ()  [unwired: 1 in, 2 out]
                  }
                  n529 = property class="DigNum (strict)"(reference=w1350, "DisabledEnum"=w1346) -> ()  [unwired: 1 in, 2 out]
                }
                frame "Probe 2" {
                  w1379 = refnum<vi> refnum  # Boolean
                  n530 = Unbundle By Name(w1382) -> ("Proble Data"=w1381:T3[])
                  n531 = To More Specific Class(target class=w1379, reference=w1378) -> (specific class reference=w1377:refnum<vi>)  [unwired: 1 in, 1 out]
                  n532 = Index Array(array=w1381, index=w1365) -> (element=w1380:T3)
                  n533 = Unbundle By Name(w1380) -> ("Active?"=w1367:bool)
                  n534 = To Variant(anything=w1367) -> (Variant=w1376:variant)
                  n535 = Select(t=T6."Enabled" ("Disabled"), s=w1367, f=T6."Disabled and Grayed Out" ("Disabled")) -> (s? t:f=w1366:T6)
                  n536 = property class="Bool"(reference=w1377, "Value"=w1376) -> ()  [unwired: 1 in, 2 out]
                  n537 = control-ref of="Probe Name 02"() -> (w1372:refnum<vi>)
                  n538 = control-ref of="Image Target 02"() -> (w1373:refnum<vi>)
                  n539 = control-ref of="Probe Sub Type 02"() -> (w1374:refnum<vi>)
                  n540 = control-ref of="Probe Cat Num 02"() -> (w1375:refnum<vi>)
                  n541 = control-ref of="Probe Concentration 02"() -> (w1370:refnum<vi>)
                  n542 = Build Array(w1372, w1373, w1374, w1375) -> (w1371:refnum<vi>[])
                  n543 = for {
                    tunnel: w1371 -> [w1384] mode=indexing
                    tunnel: w1366 -> [w1383]
                    n544 = property class="Ring (strict)"(reference=w1384, "DisabledEnum"=w1383) -> ()  [unwired: 1 in, 2 out]
                  }
                  n545 = property class="DigNum (strict)"(reference=w1370, "DisabledEnum"=w1366) -> ()  [unwired: 1 in, 2 out]
                }
                frame "Probe 3" {
                  w1399 = refnum<vi> refnum  # Boolean
                  n546 = Unbundle By Name(w1402) -> ("Proble Data"=w1401:T3[])
                  n547 = To More Specific Class(target class=w1399, reference=w1398) -> (specific class reference=w1397:refnum<vi>)  [unwired: 1 in, 1 out]
                  n548 = Index Array(array=w1401, index=w1385) -> (element=w1400:T3)
                  n549 = Unbundle By Name(w1400) -> ("Active?"=w1387:bool)
                  n550 = To Variant(anything=w1387) -> (Variant=w1396:variant)
                  n551 = Select(t=T6."Enabled" ("Disabled"), s=w1387, f=T6."Disabled and Grayed Out" ("Disabled")) -> (s? t:f=w1386:T6)
                  n552 = property class="Bool"(reference=w1397, "Value"=w1396) -> ()  [unwired: 1 in, 2 out]
                  n553 = control-ref of="Probe Name 03"() -> (w1392:refnum<vi>)
                  n554 = control-ref of="Image Target 03"() -> (w1393:refnum<vi>)
                  n555 = control-ref of="Probe Sub Type 03"() -> (w1394:refnum<vi>)
                  n556 = control-ref of="Probe Cat Num 03"() -> (w1395:refnum<vi>)
                  n557 = control-ref of="Probe Concentration 03"() -> (w1390:refnum<vi>)
                  n558 = Build Array(w1392, w1393, w1394, w1395) -> (w1391:refnum<vi>[])
                  n559 = for {
                    tunnel: w1391 -> [w1404] mode=indexing
                    tunnel: w1386 -> [w1403]
                    n560 = property class="Ring (strict)"(reference=w1404, "DisabledEnum"=w1403) -> ()  [unwired: 1 in, 2 out]
                  }
                  n561 = property class="DigNum (strict)"(reference=w1390, "DisabledEnum"=w1386) -> ()  [unwired: 1 in, 2 out]
                }
                frame "Probe 4" {
                  w1419 = refnum<vi> refnum  # Boolean
                  n562 = Unbundle By Name(w1422) -> ("Proble Data"=w1421:T3[])
                  n563 = To More Specific Class(target class=w1419, reference=w1418) -> (specific class reference=w1417:refnum<vi>)  [unwired: 1 in, 1 out]
                  n564 = Index Array(array=w1421, index=w1405) -> (element=w1420:T3)
                  n565 = Unbundle By Name(w1420) -> ("Active?"=w1407:bool)
                  n566 = To Variant(anything=w1407) -> (Variant=w1416:variant)
                  n567 = Select(t=T6."Enabled" ("Disabled"), s=w1407, f=T6."Disabled and Grayed Out" ("Disabled")) -> (s? t:f=w1406:T6)
                  n568 = property class="Bool"(reference=w1417, "Value"=w1416) -> ()  [unwired: 1 in, 2 out]
                  n569 = control-ref of="Probe Name 04"() -> (w1412:refnum<vi>)
                  n570 = control-ref of="Image Target 04"() -> (w1413:refnum<vi>)
                  n571 = control-ref of="Probe Sub Type 04"() -> (w1414:refnum<vi>)
                  n572 = control-ref of="Probe Cat Num 04"() -> (w1415:refnum<vi>)
                  n573 = control-ref of="Probe Concentration 04"() -> (w1410:refnum<vi>)
                  n574 = Build Array(w1412, w1413, w1414, w1415) -> (w1411:refnum<vi>[])
                  n575 = for {
                    tunnel: w1411 -> [w1424] mode=indexing
                    tunnel: w1406 -> [w1423]
                    n576 = property class="Ring (strict)"(reference=w1424, "DisabledEnum"=w1423) -> ()  [unwired: 1 in, 2 out]
                  }
                  n577 = property class="DigNum (strict)"(reference=w1410, "DisabledEnum"=w1406) -> ()  [unwired: 1 in, 2 out]
                }
                frame "Probe Name 01", "Probe Name 02", "Probe Name 03", "Probe Name 04" {
                  w1426 = refnum<vi> refnum  # Ring
                  n578 = Unbundle By Name(w1433) -> ("Proble Data"=w1432:T3[])
                  n579 = To More Specific Class(target class=w1426, reference=w1430) -> (specific class reference=w1429:refnum<vi>)  [unwired: 1 in, 1 out]
                  n580 = Index Array(array=w1432, index=w1425) -> (element=w1431:T3)
                  n581 = Unbundle By Name(w1431) -> ("Name.Value"=w1427:u16)
                  n582 = To Variant(anything=w1427) -> (Variant=w1428:variant)
                  n583 = property class="Ring"(reference=w1429, "Value"=w1428) -> ()  [unwired: 1 in, 2 out]
                }
                frame "Image Target 01", "Image Target 02", "Image Target 03", "Image Target 04" {
                  w1435 = refnum<vi> refnum  # Ring
                  n584 = Unbundle By Name(w1442) -> ("Proble Data"=w1441:T3[])
                  n585 = To More Specific Class(target class=w1435, reference=w1439) -> (specific class reference=w1438:refnum<vi>)  [unwired: 1 in, 1 out]
                  n586 = Index Array(array=w1441, index=w1434) -> (element=w1440:T3)
                  n587 = Unbundle By Name(w1440) -> ("Target.Value"=w1436:u16)
                  n588 = To Variant(anything=w1436) -> (Variant=w1437:variant)
                  n589 = property class="Ring"(reference=w1438, "Value"=w1437) -> ()  [unwired: 1 in, 2 out]
                }
                frame "Probe Sub Type 01", "Probe Sub Type 02", "Probe Sub Type 03", "Probe Sub Type 04" {
                  w1444 = refnum<vi> refnum  # Ring
                  n590 = Unbundle By Name(w1451) -> ("Proble Data"=w1450:T3[])
                  n591 = To More Specific Class(target class=w1444, reference=w1448) -> (specific class reference=w1447:refnum<vi>)  [unwired: 1 in, 1 out]
                  n592 = Index Array(array=w1450, index=w1443) -> (element=w1449:T3)
                  n593 = Unbundle By Name(w1449) -> ("Sub Type.Value"=w1445:u16)
                  n594 = To Variant(anything=w1445) -> (Variant=w1446:variant)
                  n595 = property class="Ring"(reference=w1447, "Value"=w1446) -> ()  [unwired: 1 in, 2 out]
                }
                frame "Probe Cat Num 01", "Probe Cat Num 02", "Probe Cat Num 03", "Probe Cat Num 04" {
                  w1453 = refnum<vi> refnum  # Ring
                  n596 = Unbundle By Name(w1460) -> ("Proble Data"=w1459:T3[])
                  n597 = To More Specific Class(target class=w1453, reference=w1457) -> (specific class reference=w1456:refnum<vi>)  [unwired: 1 in, 1 out]
                  n598 = Index Array(array=w1459, index=w1452) -> (element=w1458:T3)
                  n599 = Unbundle By Name(w1458) -> ("Cat Number.Value"=w1454:u16)
                  n600 = To Variant(anything=w1454) -> (Variant=w1455:variant)
                  n601 = property class="Ring"(reference=w1456, "Value"=w1455) -> ()  [unwired: 1 in, 2 out]
                }
                frame "Probe Concentration 01", "Probe Concentration 02", "Probe Concentration 03", "Probe Concentration 04" {
                  w1462 = refnum<vi> refnum  # Numeric
                  n602 = Unbundle By Name(w1469) -> ("Proble Data"=w1468:T3[])
                  n603 = To More Specific Class(target class=w1462, reference=w1466) -> (specific class reference=w1465:refnum<vi>)  [unwired: 1 in, 1 out]
                  n604 = Index Array(array=w1468, index=w1461) -> (element=w1467:T3)
                  n605 = Unbundle By Name(w1467) -> ("Concentration"=w1463:dbl)
                  n606 = To Variant(anything=w1463) -> (Variant=w1464:variant)
                  n607 = property class="Num"(reference=w1465, "Value"=w1464) -> ()  [unwired: 1 in, 2 out]
                }
                frame "Extra Tag 01", "Extra Tag 02", "Extra Tag 03", "Extra Tag 04", "Extra Tag 05", "Extra Tag 06" {
                  w1471 = refnum<vi> refnum  # Ring
                  n608 = Unbundle By Name(w1478) -> ("Extra Tags"=w1477:T2[])
                  n609 = To More Specific Class(target class=w1471, reference=w1475) -> (specific class reference=w1474:refnum<vi>)  [unwired: 1 in, 1 out]
                  n610 = Index Array(array=w1477, index=w1470) -> (element=w1476:T2)
                  n611 = Unbundle By Name(w1476) -> ("Value"=w1472:u16)
                  n612 = To Variant(anything=w1472) -> (Variant=w1473:variant)
                  n613 = property class="Ring"(reference=w1474, "Value"=w1473) -> ()  [unwired: 1 in, 2 out]
                }
                frame "Scavenger 01", "Scavenger 02", "Scavenger 03", "Scavenger 04", "Scavenger 05", "Scavenger 06" {
                  w1480 = refnum<vi> refnum  # Ring
                  n614 = Unbundle By Name(w1487) -> ("Scavenger Tags"=w1486:T2[])
                  n615 = To More Specific Class(target class=w1480, reference=w1484) -> (specific class reference=w1483:refnum<vi>)  [unwired: 1 in, 1 out]
                  n616 = Index Array(array=w1486, index=w1479) -> (element=w1485:T2)
                  n617 = Unbundle By Name(w1485) -> ("Value"=w1481:u16)
                  n618 = To Variant(anything=w1481) -> (Variant=w1482:variant)
                  n619 = property class="Ring"(reference=w1483, "Value"=w1482) -> ()  [unwired: 1 in, 2 out]
                }
                frame "Notes" {
                  w1491 = refnum<vi> refnum  # String
                  n620 = Unbundle By Name(w1489) -> ("Notes"=w1488:string)
                  n621 = To More Specific Class(target class=w1491, reference=w1490) -> (specific class reference=w1492:refnum<vi>)  [unwired: 1 in, 1 out]
                  n622 = property class="Str"(reference=w1492, "Value"=w1488) -> ()  [unwired: 1 in, 2 out]
                }
              }
            }
          }
          frame True {
          }
        }
      }
      event "Save New Preset": Value Change {
        n623 = event-data() -> ()  [unwired: 1 in, 1 out]
        n624 = call "Get User Input.vi"("Dialog Message"="Metadata Preset Name") -> ("User Input"=w1514:string, "Canceled?"=w1515:bool)  [unwired: 13 in]
        n625 = case shown="False" w1515 {
          tunnel: w1517 -> [w1534 _]
          tunnel: w1514 -> [w1525 _]
          tunnel: w1513 -> [w1533 w1660]
          tunnel: [w1531 w1660] -> w1512
          frame False {
            n626 = control-ref of="Preset Metadata"() -> (w1535:refnum<vi>)
            n627 = Concatenate Strings(w1525, ".json" ("string")) -> (w1537:string)
            n628 = property class="Ring (strict)"(reference=w1535) -> (reference out=w1529:refnum<vi>, "Strings []"=w1524:string[])  [unwired: 1 in, 1 out]
            n629 = Build Path(base path=w1534, name or relative path=w1537) -> (appended path=w1532:path)
            n630 = Bundle By Name(cluster=w1533, "Preset Name"=w1525) -> (w1531:T1)
            n631 = Split 1D Array(array=w1524, index=1) -> (first subarray=w1521:string[], second subarray=w1522:string[])
            n632 = Flatten To JSON(anything=w1531) -> (JSON string=w1538:string)  [unwired: 2 in, 1 out]
            n633 = Write to Text File(file (use dialog)=w1532, text=w1538) -> ()  [unwired: 2 in, 3 out]
            n634 = Build Array (concatenate)(w1522, w1525) -> (w1530:string[])
            n635 = call "Sort String Array.vi"("Array of String"=w1530) -> ("Sorted Array"=w1520:string[])  [unwired: 14 in]
            n636 = Build Array (concatenate)(w1521, w1520) -> (w1519:string[])
            n637 = for {
              tunnel: w1525 -> [w1545]
              tunnel: w1519 -> [w1543] mode=indexing
              tunnel: [w1539] -> w1527
              i -> [w1539]
              stop <- w1542 stop-if-true
              n638 = xnode "Match Regular Expression"("input string"=w1543, "regular expression"=w1545, "ignore case? (F)"=FALSE) -> ("whole match"=w1541:string)  [unwired: 3 in, 4 out]
              n639 = Not Equal?(x=w1541, y="") -> (x != y?=w1542:bool)
            }
            n640 = property class="Ring (strict)"(reference=w1529, "Strings []"=w1519) -> (reference out=w1528:refnum<vi>)  [unwired: 1 in, 1 out]
            n641 = To Unsigned Word Integer(number=w1527) -> (unsigned 16bit integer=w1526:u16)
            n642 = property class="Ring (strict)"(reference=w1528, "Value"=w1526) -> ()  [unwired: 1 in, 2 out]
          }
          frame True {
          }
        }
      }
      event "Abort": Value Change {
        n643 = event-data() -> ()  [unwired: 1 in, 1 out]
        n644 = control-ref of="This VI"() -> (w1661:refnum<vi>)
        n645 = invoke class="VI" method="Abort VI"(reference=w1661) -> ()  [unwired: 2 in, 3 out]
      }
      event "Save": Value Change {
        n646 = event-data() -> ("NewVal"=w1695:bool)  [unwired: 1 in]
        n647 = Strip Path(path=w1678) -> (stripped path=w1672:path)  [unwired: 1 out]
        n648 = Build Path(base path=w1672, name or relative path="Last File.json") -> (appended path=w1669:path)
        n649 = property on="Dirty Quit" class="Bool (strict)"("Val(Sgnl)"=TRUE ("Value (Signaling)")) -> ()  [unwired: 2 in, 2 out]
        n650 = Path To String(path=w1666) -> (string=w1670:string)
        n651 = Build Path(base path=w1672, name or relative path="Last Used.json") -> (appended path=w1692:path)
        n652 = Write to Text File(file (use dialog)=w1669, text=w1670) -> (error out=→"Last File Write Error":errorcluster)  [unwired: 2 in, 2 out]
        n653 = Flatten To JSON(anything=w1693) -> (JSON string=w1674:string, 11:w1677:errorcluster)  [unwired: 2 in]
        n654 = Write to Text File(file (use dialog)=w1692, text=w1674, error in=w1677) -> (error out=w1676:errorcluster)  [unwired: 1 in, 2 out]
        n655 = Strip Path(path=w1666) -> (stripped path=w1681:path)  [unwired: 1 out]
        n656 = Concatenate Strings(w1667, "_" ("string"), "Sample Metadata.json" ("name or relative path")) -> (w1691:string)
        n657 = call <vilib>:"Check if File or Folder Exists.vi"("error in (no error)"=w1676, "path"=w1681) -> ("error out"=w1682:errorcluster, "file or folder exists?"=w1684:bool, "dup path"=w1683:path)  [unwired: 7 in]
        n658 = case shown="False" w1684 {
          tunnel: w1683 -> [w1708 w1710]
          tunnel: [w1707 w1710] -> w1680
          tunnel: w1682 -> [w1706 w1709]
          tunnel: [w1705 w1709] -> w1675
          frame False {
            n659 = Create Folder(path (use dialog)=w1708, error in=w1706) -> (created path=w1707:path, error out=w1705:errorcluster)  [unwired: 1 in, 1 out]
          }
          frame True {
          }
        }
        n660 = Build Path(base path=w1680, name or relative path=w1691) -> (appended path=w1689:path)
        n661 = Write to Text File(file (use dialog)=w1689, text=w1674, error in=w1675) -> (error out=w1679:errorcluster)  [unwired: 1 in, 2 out]
        n662 = case shown="No Error" w1679 {
          tunnel: w1674 -> [_ w1704]
          frame No Error {
          }
          frame Error {
            w1700 = 0 items=["Desktop"=0, "Personal Documents"=5, "AppData"=26, "Local AppData"=28, "Common AppData"=35, "Program Files"=38, "Program Files Common"=43, "Common Documents"=46] ("Requested Path")
            w1701 = 0 ("HWND")
            n663 = call "Sample Metadata Get Date Time String.vi"() -> ("Date Time String"=w1697:string)  [unwired: 15 in]
            n664 = dll-call lib="shell32.dll" fn="SHGetFolderPathA"("HWND"=w1701, "nFolder"=w1700, "hToken"=w1701, "dwFlags"=w1701) -> ("pszPath"=w1702:string)  [unwired: 9 in, 2 out]
            n665 = Concatenate Strings(w1697, " Sample Metadata.json" ("string")) -> (w1696:string)
            n666 = String To Path(string=w1702) -> (path=w1703:path)
            n667 = Build Path(base path=w1703, name or relative path=w1696) -> (appended path=w1699:path)
            n668 = Write to Text File(file (use dialog)=w1699, text=w1704) -> ()  [unwired: 2 in, 3 out]
          }
        }
        n669 = Merge Errors(w1679, w1688) -> (w1687:errorcluster)
        "File Path (Dup)" <- w1666
      }
      event "Cancel": Value Change {
        n670 = event-data() -> ()  [unwired: 1 in, 6 out]
        n671 = property on="Dirty Quit" class="Bool (strict)"("Val(Sgnl)"=TRUE ("Value (Signaling)")) -> ()  [unwired: 2 in, 2 out]
      }
    }
  }
  "Write Error" <- w25
  "Canceled?" <- w24
  n672 = property class="Pnl"(reference=w16, error in=w17) -> (error out=w13:errorcluster, "Controls[]"=w15:refnum<vi>[])  [unwired: 1 out]
  n673 = To Word Integer(number=w79) -> (16bit integer=w81:i16)
  n674 = To Word Integer(number=w82) -> ()  [unwired: 1 out]
  n675 = property class="Bool (strict)"(reference=w66) -> ("Height"=w84:u32, "Top"=w85:i32)  [unwired: 1 in, 2 out]
  n676 = Unbundle By Name(w76) -> ("Left"=w78:i16, "Top"=w89:i16)
  n677 = register-events(error in=w13, w15) -> (reference out=w14:refnum<event-registration>, error out=w12:errorcluster)  [unwired: 1 in]
  n678 = To Word Integer(number=w84) -> (16bit integer=w87:i16)
  n679 = To Word Integer(number=w85) -> (16bit integer=w88:i16)
  n680 = Add(x=w78, y=w81) -> (x+y=w80:i16)
  n681 = while {
    tunnel: w14 -> [w1716]
    tunnel: w12 -> [w1715]
    tunnel: [w1713] -> w11
    stop <- w1714 stop-if-true
    n682 = event shown="[0] <Controls[]>: Value Change" {
      selector: w1716 -> [_ _]
      dyn-events: [_ _] -> w1713
      timeout: _ -> [_ _]
      tunnel: w1715 -> [_ _]
      tunnel: [FALSE ("NewVal") w1731] -> w1714
      event Value Change {
        n683 = event-data() -> ("CtlRef"=w1728:refnum<vi>)  [unwired: 1 out]
        n684 = property class="Ctl"(reference=w1728) -> ("Label.Text"=w1719:string)  [unwired: 1 in, 2 out]
        n685 = Not Equal?(x=w1719, y="Preset Metadata") -> (x != y?=w1723:bool)
        n686 = Not Equal?(x=w1719, y="Load Preset") -> (x != y?=w1721:bool)
        n687 = Not Equal?(x=w1719, y="Save New Preset") -> (x != y?=w1722:bool)
        n688 = Not Equal?(x=w1719, y="User Name") -> (x != y?=w1717:bool)
        n689 = Compound Arithmetic op=AND(w1723, w1721, w1722, w1717) -> (w1720:bool)
        n690 = case shown="True" w1720 {
          frame False {
          }
          frame True {
            n691 = control-ref of="Preset Metadata"() -> (w1729:refnum<vi>)
            n692 = property class="Ring (strict)"(reference=w1729, "Value"=u16 0) -> ()  [unwired: 1 in, 2 out]
          }
        }
      }
      event "Dirty Quit": Value Change {
        n693 = event-data() -> ("NewVal"=w1731:bool)  [unwired: 1 out]
      }
    }
  }
  n694 = Compound Arithmetic op=ADD(w89, w87, w88, i16 12 ("y")) -> (w83:i16)
  n695 = Bundle By Name(cluster=w76, "Right"=w80, "Bottom"=w83) -> (w77:T7)
  n696 = property class="VI"(reference=w75, "Front Panel.PanelBounds"=w77, "Front Panel.IsFrontmost"=TRUE ("Front Panel Window:Is Frontmost")) -> (reference out=w59:refnum<vi>)  [unwired: 1 in, 1 out]
  n697 = invoke class="VI" method="FP.Center"(reference=w59) -> ()  [unwired: 2 in, 3 out]
  n698 = Unregister For Events(event registration refnum=w11) -> ()  [unwired: 1 in, 1 out]
